vi "CaseSelect.vi"(11 "Owning VI Details":T5) -> ()   [LabVIEW 2020]
uses:
  Controls/btn-back-36x36.ctl
  Controls/btn-forward-36x36.ctl
  Controls/btn-clear-history-36x36.ctl
  Controls/btn-refresh-36x36.ctl
  <vilib>/event_ctls.llb/lveventtype.ctl
  JKI State Machine API/source/JKI SM/JKI SM.lvclass
  <vilib>/Utility/miscctls.llb/LVRectTypeDef.ctl
  JKI State Machine API/source/JKI SM/JKI SM.lvclass/JKI SM.ctl
  <vilib>/Utility/traverseref.llb/TRef TravTarget.ctl
  <vilib>/addons/_JKI Toolkits/State Machine/_JKI_lib_State_Machine.llb/Select State(s)_bool__jki_lib_state_machine.vi
  48b0ad3e-4641-4b59-aa41-8f6ed30ff61c.vi
  <userlib>/_OpenG.lib/comparison/comparison.llb/String Changed__ogtk.vi
  <userlib>/_OpenG.lib/comparison/comparison.llb/1D String Array Changed__ogtk.vi
  <userlib>/_OpenG.lib/file/file.llb/Build Path - File Names Array - path__ogtk.vi
  <vilib>/regexp/Match Regular Expression.xnode
  <userlib>/_OpenG.lib/comparison/comparison.llb/openg_comparison__ogtk.lvlib
  <userlib>/_OpenG.lib/time/time.llb/openg_time.lvlib
  <userlib>/_OpenG.lib/file/file.llb/openg_file.lvlib
panel:
  in  "Refresh":T1
  in  "Clear History":T2
  in  "Forward":T3
  in  "Back":T4
  in  "Search Icon":bool
  in  "Clear Search":bool
  in  "Search":string
  in  "Add macro":bool
  in  "Tree":string(tree) caption="Cases"
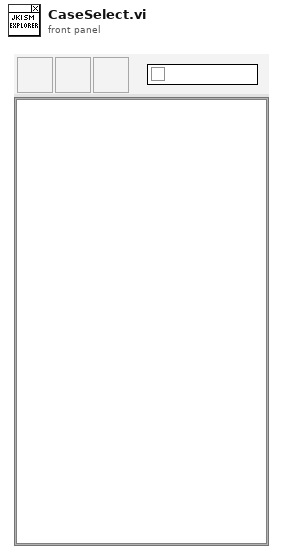
[diagram p1: front panel]
types:
  T1 = typedef "btn-refresh-36x36.ctl" = bool
  T2 = typedef "btn-clear-history-36x36.ctl" = bool
  T3 = typedef "btn-forward-36x36.ctl" = bool
  T4 = typedef "btn-back-36x36.ctl" = bool
  T5 = cluster{"App.ContextName":string, "VI.Name":string, "Object UID":i32}
  T6 = enum32{"Invalid", "Standard", "Closed", "Hidden", "Minimized", "Maximized"}
  T7 = typedef "lveventtype.ctl" = enum32{"Null", "Timeout", "Annotation Menu Selection", "Annotation Menu Selection?", "App Instance Close", "App Instance Close?", "Autoscale Range Change", "Bookmark Info Change", "Cell Edit", "Cell Edit?", "Cursor Grab", "Cursor Grab?", "Cursor Menu Selection", "Cursor Menu Selection?", "Cursor Move", "Cursor Release", "Data Change", "Direction Change", "Display State Change", "Drag Ended", "Drag Enter", "Drag Leave", "Drag Over", "Drag Source Update", "Drag Starting", "Drag Starting?", "Drop", "Exec State Change", "Key Down", "Key Down?", "Key Repeat", "Key Repeat?", "Key Up", "Listbox Double Click", "Menu Activation?", "Menu Selection (App)", "Menu Selection? (App)", "Menu Selection (User)", "Mouse Down", "Mouse Down?", "Mouse Enter", "Mouse Leave", "Mouse Move", "Mouse Up", "Mouse Wheel", "NI Security User Change (App)", "Pane Size", "Panel Close", "Panel Close?", "Panel Resize", "Plot Attribute Change", "Scale Range Change", "Shortcut Menu Activation?", "Shortcut Menu Selection (App)", "Shortcut Menu Selection? (App)", "Shortcut Menu Selection (User)", "Tree Double Click", "Tree Drag", "Tree Drag?", "Tree Drop", "Tree Drop?", "Tree Item Close", "Tree Item Close?", "Tree Item Open", "Tree Item Open?", "User Event", "Value Change"}
  T8 = enum32{"invalid app kind", "Development System", "Run Time System", "Student Edition", "Embedded LabVIEW", "Evaluation", "Custom"}
  T9 = typedef "TRef TravTarget.ctl" = enum16{"FP", "BD", "Other"}
  T10 = typedef "LVPoint32TypeDef.ctl" = cluster{"Horizontal":i32, "Vertical":i32}
  T11 = typedef "LVNodeAndColumnTypeDef.ctl" = cluster{"Node":string, "Column":i32}
  T12 = typedef "LVRectTypeDef.ctl" = cluster{"Left":i16, "Top":i16, "Right":i16, "Bottom":i16}
  T13 = cluster{"OpenCategoryFrames":refnum<vi>[], "Frames[]":refnum<vi>[], "Core":cluster{"Current VI Reference":refnum<vi>, "Close Panel on Exit?":bool}, "Indent?":bool, "InBounds":bool, "Activating":bool, "FrameNames":string[], "tag":string, "Top Row Tag":string, "TreeSectHdrs":string, "SectHdr":string, "CaseStrVIName":string, "TempString":string, "DisplayedItems":i32, "SelectedCase":u32, "Display:Primary Workspace":T12, "Tree":refnum<vi>, "StructRef":refnum<vi>, "CaseStrVI Ref":refnum<vi>, "Ctrl?":bool, "NavHist":refnum<vi>[], "NavIndex":i32, "Undo Transaction":bool, "Top Row Index":i32, "JKI SM":refnum<class "JKI SM.lvclass">, "Num Event Frames":i32, "Error During Startup":bool}
  T14 = cluster{"Current VI Reference":refnum<vi>, "Close Panel on Exit?":bool}
  T15 = enum8{"Enabled", "Disabled", "Disabled and Grayed Out"}
  T16 = enum32{"Bad", "Idle", "Run top level", "Running"}
  T17 = typedef "StructureTypes.ctl" = enum16{"CaseStructure", "EventStructure"}
  T18 = cluster{"StringConstant":refnum<vi>, "Structure":string, "Frame Name":string, "State Call":string, "UID":dbl}[]
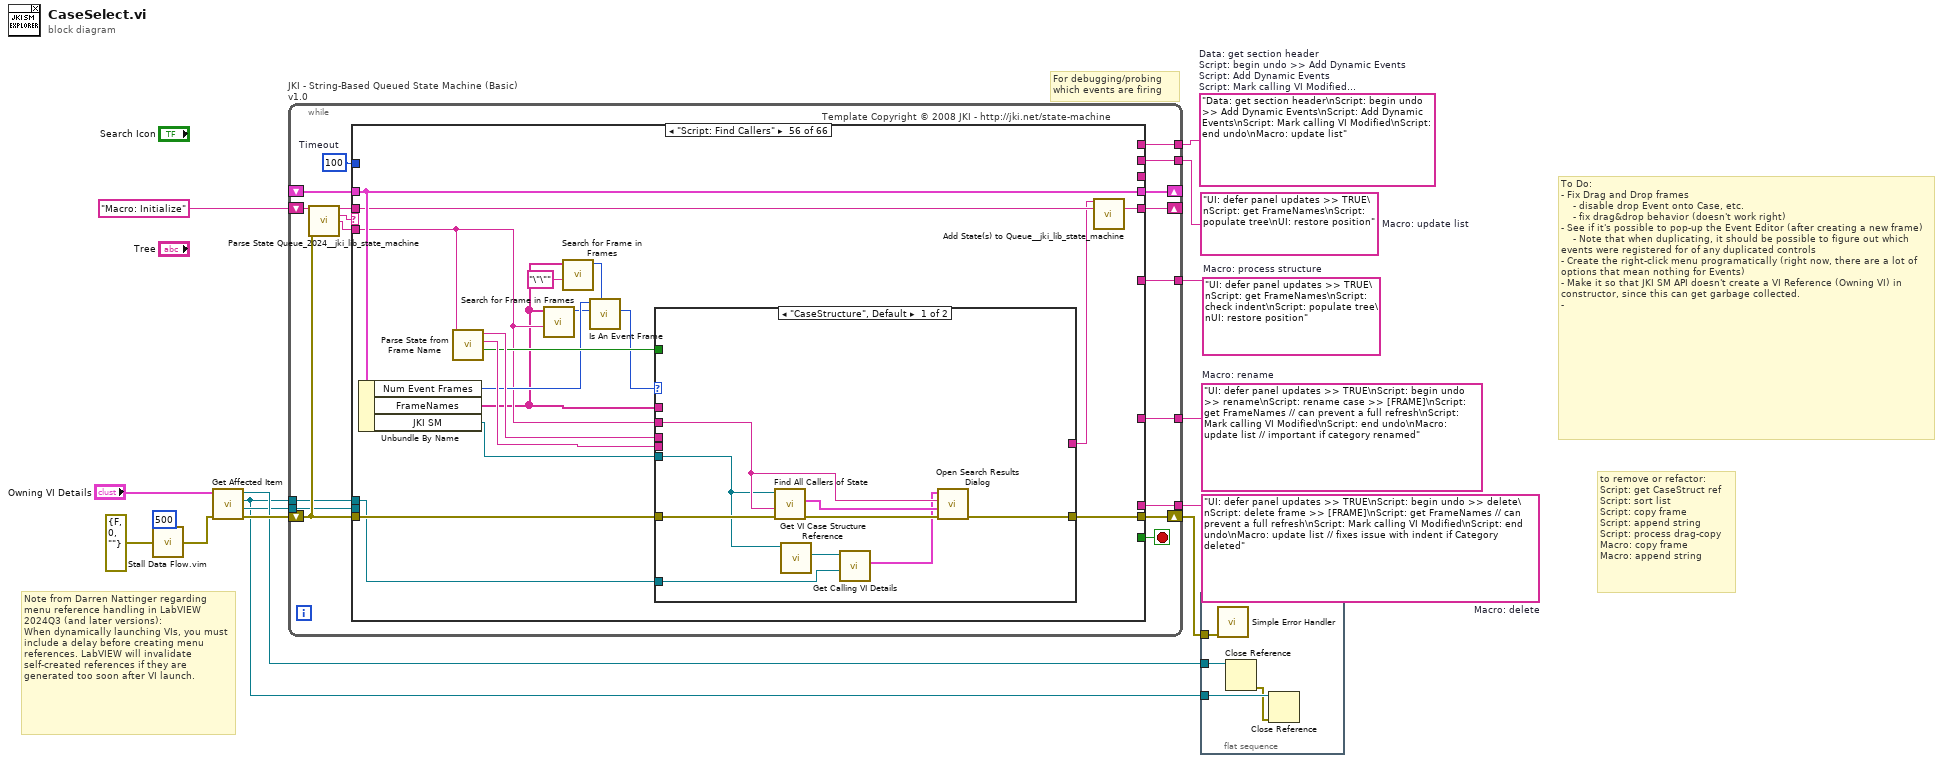
[diagram p0: block diagram]
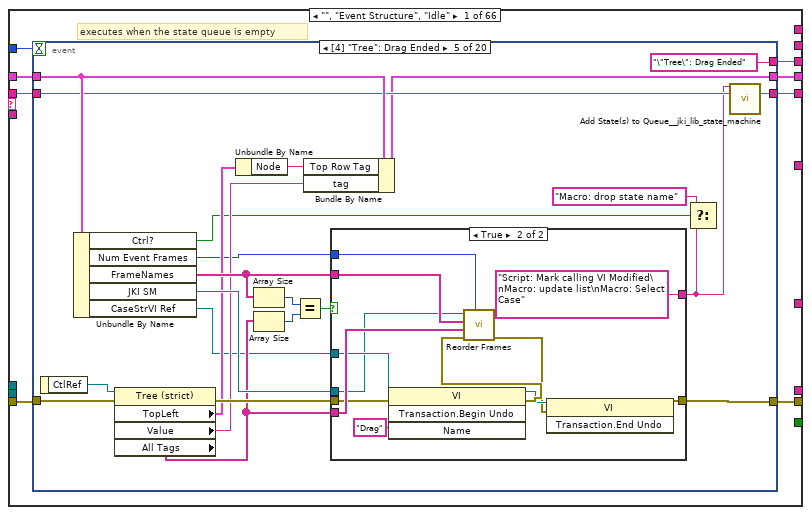
[diagram p2: hidden frame]
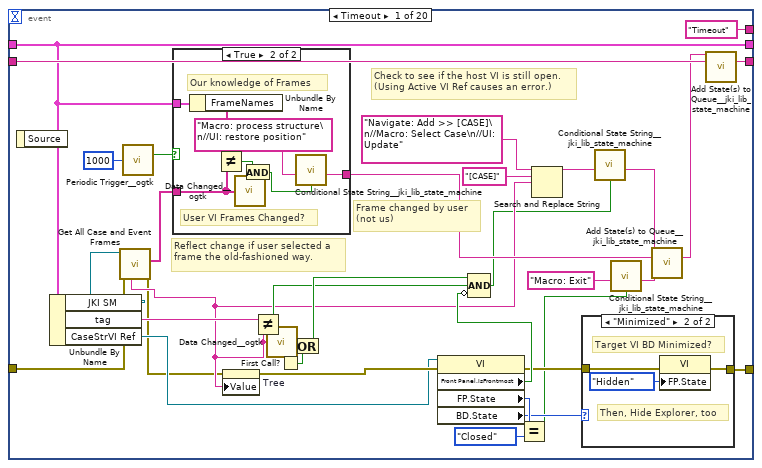
[diagram p3: hidden frame]
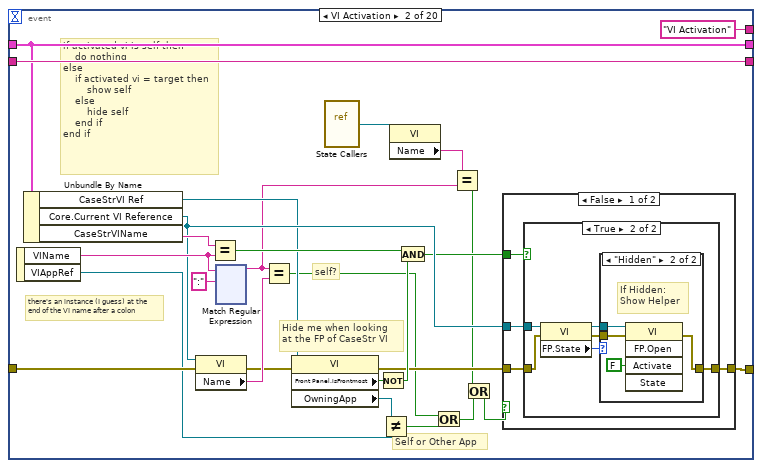
[diagram p6: hidden frame]
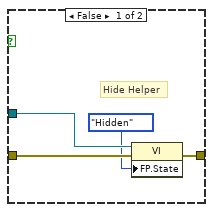
[diagram p7: hidden frame]
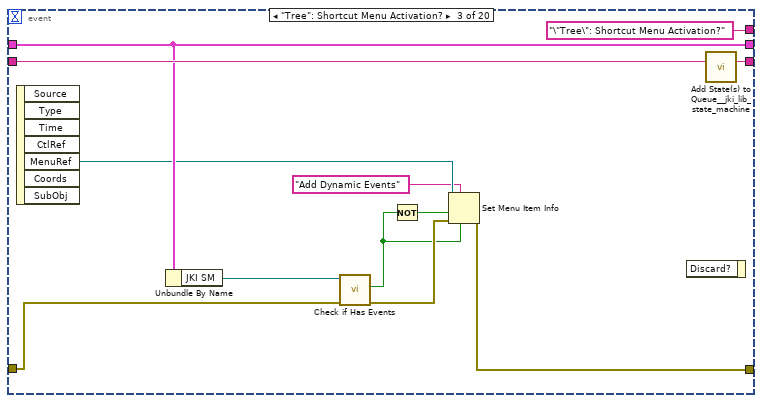
[diagram p10: hidden frame]
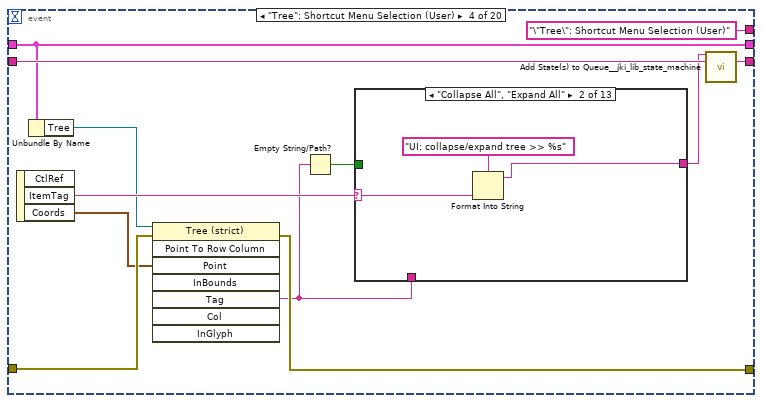
[diagram p11: hidden frame]
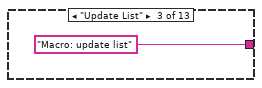
[diagram p13: hidden frame]
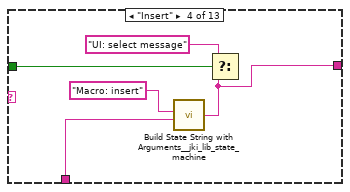
[diagram p14: hidden frame]
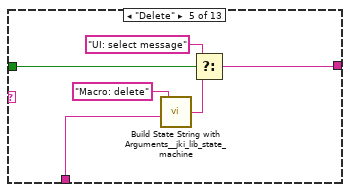
[diagram p15: hidden frame]
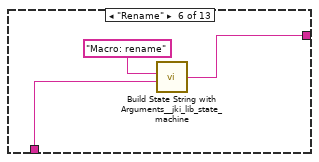
[diagram p16: hidden frame]
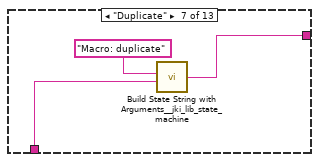
[diagram p17: hidden frame]
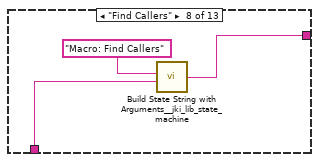
[diagram p18: hidden frame]
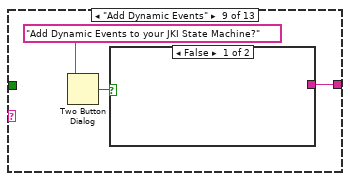
[diagram p19: hidden frame]
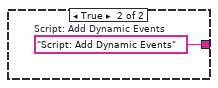
[diagram p20: hidden frame]
diagram:
  w9 = "Data: get section header\nScript: begin undo >> Add Dynamic Events\nScript: Add Dynamic Events\nScript: Mark calling VI Modified\nScript: end undo\nMacro: update list"  # Data: get section header Script: begin undo >> Add Dynamic Events Script: Add Dynamic Events Script: Mark calling VI Modified Script: end undo Macro: update list
  w10 = "UI: defer panel updates >> TRUE\nScript: get FrameNames\nScript: populate tree\nUI: restore position"  # Macro: update list
  w12 = "UI: defer panel updates >> TRUE\nScript: begin undo >> delete\nScript: delete frame >> [FRAME]\nScript: get FrameNames // can prevent a full refresh\nScript: Mark calling VI Modified\nScript: end undo\nMacro: update list // fixes issue with indent if Category deleted"  # Macro: delete
  w13 = "UI: defer panel updates >> TRUE\nScript: begin undo >> rename\nScript: rename case >> [FRAME]\nScript: get FrameNames // can prevent a full refresh\nScript: Mark calling VI Modified\nScript: end undo\nMacro: update list // important if category renamed"  # Macro: rename
  w14 = "UI: defer panel updates >> TRUE\nScript: get FrameNames\nScript: check indent\nScript: populate tree\nUI: restore position"  # Macro: process structure
  # "Note from Darren Nattinger regarding menu reference handling in LabVIEW 2024Q3 (and later versions):\nWhen dynamically launching VIs, you must include a delay before creating menu references. LabVIEW will invalidate self-created references if they are generated too soon after VI launch."
  # "to remove or refactor:\nScript: get CaseStruct ref\nScript: sort list\nScript: copy frame\nScript: append string\nScript: process drag-copy\nMacro: copy frame\nMacro: append string"
  # "For debugging/probing which events are firing"
  # "To Do:\n- Fix Drag and Drop frames\n    - disable drop Event onto Case, etc.\n    - fix drag&drop behavior (doesn't work right)\n- See if it's possible to pop-up the Event Editor (after creating a new frame)\n    - Note that when duplicating, it should be possible to figure out which events were registered for of any duplicated controls\n- Create the right-click menu programatically (right now, there are a lot of options that mean nothing for Events)\n- Make it so that JKI SM API doesn't create a VI Reference (Owning VI) in constructor, since this can get garbage collected.\n-"
  n1 = call "Stall Data Flow.vim"("value in"=errorcluster {"status"=FALSE, "code"=0, "source"=""} ("error in (no error)"), "milliseconds to wait"=u32 500) -> ("value out"=w5:errorcluster)  [unwired: 1 out]
  n2 = call "Get Affected Item.vi"("error in (no error)"=w5, "Owning VI Details"="Owning VI Details") -> ("error out"=w7:errorcluster, "GObject"=w2:refnum<vi>, "Owning VI"=w1:refnum<vi>, "Application"=w6:refnum<vi>)  [unwired: 6 in]
  n3 = while "JKI - String-Based Queued State Machine (Basic) v1.0" {
    shift-right: [w30] -> _
    shift-left: _ -> [w29]
    shift-right: [w33] -> w11
    shift-left: w7 -> [w21]
    shift-right: [w32] -> _
    shift-left: "Macro: Initialize" -> [w22]
    tunnel: w14 -> [w27]
    tunnel: w13 -> [w26]
    tunnel: w12 -> [w25]
    tunnel: w10 -> [w24]
    tunnel: w9 -> [w23]
    tunnel: w2 -> [w17]
    tunnel: w1 -> [w16]
    stop <- w31 stop-if-true
    w28 = 100  # Timeout
    # "Template Copyright © 2008 JKI - http://jki.net/state-machine"
    n4 = call <vilib>:"Parse State Queue_2024__jki_lib_state_machine.vi"("State Queue"=w22, "Error In (no error)"=w21) -> ("Remaining States"=w18:string, "Current State"=w19:string, "Arguments"=w20:string)  [unwired: 11 in]
    n5 = case shown="\"Script: Find Callers\"" w19 {
      selector: w19 -> [_ _ w578 _ _ _ _ _ _ _ _ _ _ _ _ _ _ _ _ _ _ _ _ _ _ _ _ _ _ _ _ _ _ _ _ _ _ _ _ _ _ _ _ _ _ _ _ _ _ _ _ _ _ _ _ _ _ _ _ _ _ _ _ _ _ _]
      tunnel: w18 -> [w41 w574 w577 w587 w606 _ w632 w636 w657 w698 w715 w728 w731 w739 w755 w757 w799 w809 w827 w852 w881 w893 w895 w902 w905 w913 w923 w942 w945 w951 w955 w966 w974 w979 w988 w992 w997 w1007 w1014 w1015 w1028 w1045 w1046 w1059 w1073 w1093 w1094 w1133 w1188 w1209 w1214 w1223 w1305 w1351 w1398 w1456 w1485 w1511 w1546 w1569 w1578 w1588 w1596 w1611 w1661 w1670]
      tunnel: w20 -> [_ _ _ _ _ w617 _ _ _ _ _ _ _ _ _ w756 _ w812 _ w854 _ _ _ _ _ w908 w919 w938 _ _ _ w959 w971 _ w985 _ _ w1004 _ _ w1018 _ _ w1056 _ _ _ _ _ _ _ w1217 w1299 w1340 w1390 w1445 w1478 _ w1535 _ _ _ _ _ _ _]
      tunnel: w29 -> [w39 w575 w580 w590 w607 w624 w635 w637 _ w697 w713 w729 w732 w740 w753 w759 w798 w814 w831 w850 w880 w892 w896 w899 w906 w914 w924 w935 w946 w949 w957 w960 w975 w980 w989 w994 w999 w1009 w1011 w1016 w1026 w1042 w1047 w1057 w1072 w1091 w1102 w1116 w1187 w1208 w1213 w1225 w1308 w1344 w1400 w1458 w1486 w1521 w1551 w1570 w1577 w1587 w1595 w1621 w1660 w1669]
      tunnel: [w38 w576 w582 w596 w608 w625 w634 w638 w641 w699 w714 w722 w733 w738 w754 w760 w796 w815 w832 w856 w879 w894 w897 w900 w907 w915 w917 w937 w947 w952 w956 w962 w969 w977 w983 w993 w998 w1008 w1012 w1017 w1022 w1037 w1048 w1058 w1069 w1087 w1095 w1128 w1186 w1207 w1211 w1219 w1307 w1352 w1399 w1457 w1475 w1515 w1537 w1568 w1574 w1584 w1592 w1614 w1655 w1665] -> w33
      tunnel: w21 -> [w37 w576 w581 w596 w608 w619 w634 w638 w651 w699 w714 w727 w733 w738 w754 w761 w797 w816 w833 w855 w882 w894 w897 w900 w907 w915 w918 w933 w947 w952 w956 w963 w970 w977 w984 w993 w998 w1008 w1012 w1017 w1020 w1038 w1048 w1052 w1070 w1078 w1096 w1134 w1177 w1206 w1212 w1226 w1297 w1349 w1394 w1452 w1476 w1519 w1536 w1568 w1576 w1586 w1594 w1620 w1657 w1668]
      tunnel: [w40 w574 w577 w587 w606 w621 w632 w636 w657 w698 w715 w728 w731 w739 w755 w757 w799 w808 w826 w851 w881 w893 w895 w901 w904 w912 w922 w941 w944 w950 w954 w965 w973 w978 w987 w991 w996 w1006 w1013 w1015 w1028 w1045 w1046 w1059 w1073 w1092 w1094 w1133 w1188 w1209 w1214 w1222 w1304 w1351 w1397 w1455 w1484 w1510 w1545 w1569 w1578 w1588 w1596 w1610 w1661 w1670] -> w32
      tunnel: [_ _ _ _ _ _ TRUE _ _ _ _ _ _ _ _ _ _ _ _ _ _ _ _ _ _ _ _ _ _ _ _ _ _ _ _ _ _ _ _ _ _ _ _ _ _ _ _ _ _ _ _ _ _ _ _ _ _ _ _ _ _ _ _ _ _ _] -> w31
      tunnel: [w36 w575 w580 w597 w607 w624 w635 w637 w679 w696 w709 w729 w732 w740 w753 w759 w798 w814 w828 w849 w880 w892 w896 w899 w906 w914 w924 w935 w946 w949 w957 w960 w975 w980 w989 w994 w999 w1009 w1011 w1016 w1027 w1041 w1047 w1055 w1071 w1090 w1101 w1132 w1183 w1208 w1213 w1225 w1308 w1343 w1400 w1458 w1486 w1509 w1541 w1570 w1573 w1587 w1591 w1621 w1660 w1669] -> w30
      tunnel: w28 -> [w35 _ _ _ _ _ _ _ _ _ _ _ _ _ _ _ _ _ _ _ _ _ _ _ _ _ _ _ _ _ _ _ _ _ _ _ _ _ _ _ _ _ _ _ _ _ _ _ _ _ _ _ _ _ _ _ _ _ _ _ _ _ _ _ _ _]
      tunnel: w27 -> [_ _ _ _ _ _ _ _ _ _ _ _ _ _ _ _ _ _ _ _ _ _ _ _ w903 _ _ _ _ _ _ _ _ _ _ _ _ _ _ _ _ _ _ _ _ _ _ _ _ _ _ _ _ _ _ _ _ _ _ _ _ _ _ _ _ _]
      tunnel: w26 -> [_ _ _ _ _ _ _ _ _ _ _ _ _ _ _ _ _ _ _ _ _ _ _ _ _ _ _ _ _ _ _ w958 _ _ _ _ _ _ _ _ _ _ _ _ _ _ _ _ _ _ _ _ _ _ _ _ _ _ _ _ _ _ _ _ _ _]
      tunnel: w25 -> [_ _ _ _ _ _ _ _ _ _ _ _ _ _ _ _ _ _ _ _ _ _ _ _ _ _ w916 _ _ _ _ _ _ _ _ _ _ _ _ _ _ _ _ _ _ _ _ _ _ _ _ _ _ _ _ _ _ _ _ _ _ _ _ _ _ _]
      tunnel: w24 -> [_ _ _ _ _ _ _ _ _ _ _ _ _ _ _ _ _ _ _ _ _ _ _ _ _ _ _ _ w943 _ _ _ _ _ _ _ _ _ _ _ _ _ _ _ _ _ _ _ _ _ _ _ _ _ _ _ _ _ _ _ _ _ _ _ _ _]
      tunnel: w23 -> [_ _ _ _ _ _ _ _ _ _ _ _ _ _ _ _ _ _ _ _ _ _ _ _ _ _ _ _ _ _ _ _ _ w976 _ _ _ _ _ _ _ _ _ _ _ _ _ _ _ _ _ _ _ _ _ _ _ _ _ _ _ _ _ _ _ _]
      tunnel: [w34 _ _ _ _ _ _ _ _ _ _ _ _ _ _ _ _ _ _ _ _ _ _ _ _ _ _ _ _ _ _ _ _ _ _ _ _ _ _ _ _ _ _ _ _ _ _ _ _ _ _ _ _ _ _ _ _ _ _ _ _ _ _ _ _ _] -> _
      tunnel: w17 -> [_ _ _ _ _ _ _ _ w640 _ _ _ _ _ _ _ _ _ _ _ _ _ _ _ _ _ _ _ _ _ _ _ _ _ _ _ _ _ _ _ _ _ _ _ _ _ _ _ _ _ _ _ _ _ _ _ _ _ _ _ _ _ _ _ _ _]
      tunnel: w16 -> [_ _ _ _ _ _ _ _ w639 _ _ _ _ _ _ _ _ _ _ _ _ _ _ _ _ _ _ _ _ _ _ _ _ _ _ _ _ _ _ _ _ _ _ _ _ _ _ _ _ _ _ _ _ _ _ w1441 _ _ _ _ _ _ _ _ _ _]
      frame "", "Event Structure", "Idle" {
        # "executes when the state queue is empty"
        n6 = event shown="[4] \"Tree\": Drag Ended" {
          selector: _ -> [_ _ _ _ _ _ _ _ _ _ _ _ _ _ _ _ _ _ _ _]
          dyn-events: _ -> [_ _ _ _ _ _ _ _ _ _ _ _ _ _ _ _ _ _ _ _]
          timeout: w35 -> [_ _ _ _ _ _ _ _ _ _ _ _ _ _ _ _ _ _ _ _]
          tunnel: w41 -> [w75 w114 w257 w267 w319 w346 w356 w363 w397 w442 w458 w494 w497 w506 w515 w536 w555 w559 w566 w573]
          tunnel: [w74 w114 w256 w266 w318 w345 w356 w362 w396 w442 w457 w494 w496 w505 w514 w535 w554 w560 w566 w572] -> w40
          tunnel: w39 -> [w57 w112 w255 w264 w321 w347 w355 w360 w391 w439 w459 w492 w500 w509 w518 w548 w552 w561 w564 w570]
          tunnel: [w48 w110 w250 w260 w308 w343 w351 w364 w394 w435 w460 w493 w499 w508 w517 w527 w556 w562 w563 w571] -> w38
          tunnel: w37 -> [w53 w102 w254 w269 w323 w343 w352 w365 w394 w436 w460 w493 w499 w508 w517 w524 w556 w562 w563 w571]
          tunnel: [w57 w112 w255 w264 w312 w344 w350 w360 w390 w439 w455 w492 w500 w509 w518 w549 w552 w561 w564 w570] -> w36
          tunnel: ["Timeout" ("State(s) in Front (\"\")") "VI Activation" ("State(s) in Front (\"\")") "\"Tree\": Shortcut Menu Activation?" ("State(s) in Front (\"\")") "\"Tree\": Shortcut Menu Selection (User)" ("State(s) in Front (\"\")") "\"Tree\": Drag Ended" ("State(s) in Front (\"\")") "\"Tree\": Value Change" ("State(s) in Front (\"\")") "\"Tree\": Mouse Down" ("State(s) in Front (\"\")") "\"Tree\": Mouse Up" ("State(s) in Front (\"\")") "\"Tree\": Item Close" ("State(s) in Front (\"\")") "\"Tree\": Mouse Move" ("State(s) in Front (\"\")") "Key Down?" ("State(s) in Front (\"\")") "Mouse Leave" ("State(s) in Front (\"\")") "Panel Resize" ("State(s) in Front (\"\")") "\"Search\": Value Change" ("State(s) in Front (\"\")") "\"Clear Search\": Value Change" ("State(s) in Front (\"\")") "\"Back\", \"Forward\": Value Change" ("State(s) in Front (\"\")") "\"Clear History\": Value Change" ("State(s) in Front (\"\")") "\"Refresh\": Value Change" ("State(s) in Front (\"\")") "\"Add macro\": Value Change" ("State(s) in Front (\"\")") "Panel Close?" ("State(s) in Front (\"\")")] -> w34
          event Timeout {
            # "Frame changed by user\n(not us)"
            # "Reflect change if user selected a frame the old-fashioned way."
            # "Check to see if the host VI is still open.\n(Using Active VI Ref causes an error.)"
            n7 = event-data() -> ()  [unwired: 2 out]
            n8 = Unbundle By Name(w57) -> ("JKI SM"=w56:refnum<class "JKI SM.lvclass">, "tag"=w70:string, "CaseStrVI Ref"=w60:refnum<vi>)
            n9 = call "Get All Case and Event Frames.vi"("error in (no error)"=w53, "JKI SM in"=w56) -> ("error out"=w52:errorcluster, "Frame Names"=w55:string[], "Visible Frame Name"=w54:string)  [unwired: 1 in, 6 out]
            n10 = call <userlib>:"Periodic Trigger__ogtk.vi"("time (ms)"=u32 1000) -> ("Triggered"=w62:bool)  [unwired: 12 in, 2 out]
            n11 = case shown="True" w62 {
              tunnel: [_ w80] -> w61
              tunnel: w57 -> [_ w87]
              tunnel: w55 -> [_ w83]
              frame False {
              }
              frame True {
                # "Our knowledge of Frames"
                # "User VI Frames Changed?"
                n12 = Unbundle By Name(w87) -> ("FrameNames"=w86:string[])
                n13 = Not Equal?(x=w86, y=w83) -> (x != y?=w85:bool)
                n14 = call-poly <userlib>:"Data Changed__ogtk.vi"("1D String Array"=w83) -> ("Changed"=w84:bool)
                n15 = And(x=w85, y=w84) -> (x .and. y?=w81:bool)
                n16 = call <vilib>:"Conditional State String__jki_lib_state_machine.vi"("Do State(s)?"=w81, "State"="Macro: process structure\n//UI: restore position") -> ("State Out"=w80:string)  [unwired: 7 in]
              }
            }
            n17 = property on="Tree" class="Tree (strict)"(error in=w52, "Value"=w54) -> (error out=w71:errorcluster)  [unwired: 1 in, 1 out]
            n18 = Not Equal?(x=w70, y=w54) -> (x != y?=w58:bool)
            n19 = call-poly <userlib>:"Data Changed__ogtk.vi"("String"=w54) -> ("Changed"=w65:bool)
            n20 = First Call?() -> (First Call?: T/F=w66:bool)
            n21 = Or(x=w65, y=w66) -> (x .or. y?=w64:bool)
            n22 = property class="VI"(reference=w60, error in=w71) -> (error out=w49:errorcluster, "Front Panel.IsFrontmost"=w59:bool, "FP.State"=w73:T6, "BD.State"=w50:T6)  [unwired: 1 out]
            n23 = Compound Arithmetic op=AND(w64, w58, invert w59) -> (w46:bool)
            n24 = Equal?(x=w73, y=T6."Closed" ("Front Panel Window:State")) -> (x = y?=w43:bool)
            n25 = Search and Replace String(input string="Navigate: Add >> [CASE]\n//Macro: Select Case\n//UI: Update" ("State(s) in Front (\"\")"), search string="[CASE]", replace string=w54) -> (result string=w47:string)  [unwired: 5 in, 3 out]
            n26 = case shown="\"Minimized\"" w50 {
              tunnel: w49 -> [w76 w79]
              tunnel: [w76 w78] -> w48
              frame Default {
              }
              frame "Minimized" {
                # "Then, Hide Explorer, too"
                # "Target VI BD Minimized?"
                n27 = property class="VI"(error in=w79, "FP.State"=T6."Hidden" ("Front Panel Window:State")) -> (error out=w78:errorcluster)  [unwired: 1 in, 1 out]
              }
            }
            n28 = call <vilib>:"Conditional State String__jki_lib_state_machine.vi"("Do State(s)?"=w46, "State"=w47) -> ("State Out"=w45:string)  [unwired: 7 in]
            n29 = call <vilib>:"Conditional State String__jki_lib_state_machine.vi"("Do State(s)?"=w43, "State"="Macro: Exit") -> ("State Out"=w42:string)  [unwired: 7 in]
            n30 = call <vilib>:"Add State(s) to Queue__jki_lib_state_machine.vi"("State(s) in Front (\"\")"=w45, "State(s) in (\"\")"=w61, "State(s) at Back (\"\")"=w42) -> ("States Out"=w67:string)  [unwired: 12 out]
            n31 = call <vilib>:"Add State(s) to Queue__jki_lib_state_machine.vi"("State(s) in Front (\"\")"=w67, "State(s) in (\"\")"=w75) -> ("States Out"=w74:string)  [unwired: 1 in, 12 out]
          }
          event VI Activation {
            # "Self or Other App"
            # "self?"
            # "Hide me when looking\nat the FP of CaseStr VI"
            # "there's an instance (I guess) at the\nend of the VI name after a colon"
            # "if activated vi is self then\n    do nothing\nelse\n    if activated vi = target then\n        show self\n    else\n        hide self\n    end if\nend if"
            n32 = event-data() -> ("VIName"=w107:string, "VIAppRef"=w97:refnum<vi>)  [unwired: 1 out]
            n33 = Unbundle By Name(w112) -> ("CaseStrVI Ref"=w100:refnum<vi>, "Core.Current VI Reference"=w106:refnum<vi>, "CaseStrVIName"=w113:string)
            n34 = property class="VI"(reference=w106, error in=w102) -> (error out=w101:errorcluster, "Name"=w108:string)  [unwired: 1 out]
            n35 = Equal?(x=w113, y=w107) -> (x = y?=w111:bool)
            n36 = xnode "Match Regular Expression"("input string"=w107, "regular expression"=":") -> ("before match"=w92:string)  [unwired: 3 in, 5 out]
            n37 = Equal?(x=w92, y=w108) -> (x = y?=w95:bool)
            n38 = property class="VI"(reference=w100, error in=w101) -> (error out=w103:errorcluster, "Front Panel.IsFrontmost"=w105:bool, "OwningApp"=w98:refnum<vi>)  [unwired: 1 out]
            n39 = vi-ref "State Callers.vi"() -> (w94:refnum<vi>)
            n40 = Not(x=w105) -> (.not. x?=w104:bool)
            n41 = Not Equal?(x=w98, y=w97) -> (x != y?=w96:bool)
            n42 = property class="VI"(reference=w94) -> ("Name"=w93:string)  [unwired: 1 in, 2 out]
            n43 = And(x=w111, y=w104) -> (x .and. y?=w99:bool)
            n44 = Or(x=w95, y=w96) -> (x .or. y?=w90:bool)
            n45 = Equal?(x=w93, y=w92) -> (x = y?=w91:bool)
            n46 = Or(x=w91, y=w90) -> (x .or. y?=w89:bool)
            n47 = case shown="False" w89 {
              tunnel: w103 -> [w118 w134]
              tunnel: [w116 w134] -> w110
              tunnel: w106 -> [w117 _]
              tunnel: w99 -> [w115 _]
              frame False {
                n48 = case shown="True" w115 {
                  tunnel: w118 -> [w122 w127]
                  tunnel: w117 -> [w121 w128]
                  tunnel: [w120 w125] -> w116
                  frame False {
                    # "Hide Helper"
                    n49 = property class="VI"(reference=w121, error in=w122, "FP.State"=T6."Hidden" ("Front Panel Window:State")) -> (error out=w120:errorcluster)  [unwired: 1 out]
                  }
                  frame True {
                    n50 = property class="VI"(reference=w128, error in=w127) -> (reference out=w124:refnum<vi>, error out=w123:errorcluster, "FP.State"=w126:T6)
                    n51 = case shown="\"Hidden\"" w126 {
                      tunnel: [w129 w133] -> w125
                      tunnel: w124 -> [_ w132]
                      tunnel: w123 -> [w129 w131]
                      frame Default {
                      }
                      frame "Hidden" {
                        # "If Hidden:\nShow Helper"
                        n52 = invoke class="VI" method="FP.Open"(reference=w132, error in=w131, "Activate"=FALSE ("Activate?")) -> (error out=w133:errorcluster)  [unwired: 2 in, 4 out]
                      }
                    }
                  }
                }
              }
              frame True {
              }
            }
          }
          event "Tree": Shortcut Menu Activation? {
            n53 = event-data() -> ("MenuRef"=w252:refnum<k9>)  [unwired: 7 out]
            n54 = Unbundle By Name(w255) -> ("JKI SM"=w247:refnum<class "JKI SM.lvclass">)
            n55 = call "Check if Has Events.vi"("error in (no error)"=w254, "JKI SM in"=w247) -> ("error out"=w251:errorcluster, "Has Dyanamic Events?"=w249:bool)  [unwired: 7 in, 1 out]
            n56 = Not(x=w249) -> (.not. x?=w253:bool)
            n57 = Set Menu Item Info(6:w249, 7:"Add Dynamic Events" ("item name"), 8:w251, 9:w253, 11:w252) -> (0:w250:errorcluster)  [unwired: 2 in, 1 out]
            n58 = event-data() -> ()  [unwired: 2 in, 1 out]
            n59 = call <vilib>:"Add State(s) to Queue__jki_lib_state_machine.vi"("State(s) in (\"\")"=w257) -> ("States Out"=w256:string)  [unwired: 2 in, 12 out]
          }
          event "Tree": Shortcut Menu Selection (User) {
            n60 = event-data() -> ("ItemTag"=w268:string, "Coords"=w261:T10)  [unwired: 2 out]
            n61 = Unbundle By Name(w264) -> ("Tree"=w263:refnum<vi>)
            n62 = invoke class="Tree (strict)" method="Point To Row Column"(reference=w263, error in=w269, "Point"=w261) -> (error out=w260:errorcluster, "Tag"=w259:string)  [unwired: 5 in, 6 out]
            n63 = Empty String/Path?(string/path=w259) -> (empty?=w262:bool)
            n64 = case shown="\"Collapse All\", \"Expand All\"" w268 {
              selector: w268 -> [_ w271 _ _ _ _ _ _ _ _ _ _ _]
              tunnel: [_ w270 "Macro: update list" w274 w282 w285 w288 w291 w296 "Macro: sort list" _ w299 _] -> w265
              tunnel: w262 -> [_ _ _ w278 w284 _ _ _ _ _ _ _ _]
              tunnel: w259 -> [_ _ _ w275 w280 w287 w290 w293 _ _ _ _ w300]
              frame Default {
              }
              frame "Collapse All", "Expand All" {
                n65 = Format Into String(format string="UI: collapse/expand tree >> %s", w271) -> (resulting string=w270:string)  [unwired: 2 in, 1 out]
              }
              frame "Update List" {
              }
              frame "Insert" {
                n66 = call <vilib>:"Build State String with Arguments__jki_lib_state_machine.vi"("Arguments (\"\")"=w275, "State"="Macro: insert") -> ("State with Arguments"=w274:string)  [unwired: 4 in]
                n67 = Select(t="UI: select message", s=w278, f=w274) -> ()  [unwired: 1 out]
              }
              frame "Delete" {
                n68 = call <vilib>:"Build State String with Arguments__jki_lib_state_machine.vi"("Arguments (\"\")"=w280, "State"="Macro: delete") -> ("State with Arguments"=w279:string)  [unwired: 4 in]
                n69 = Select(t="UI: select message", s=w284, f=w279) -> (s? t:f=w282:string)
              }
              frame "Rename" {
                n70 = call <vilib>:"Build State String with Arguments__jki_lib_state_machine.vi"("Arguments (\"\")"=w287, "State"="Macro: rename") -> ("State with Arguments"=w285:string)  [unwired: 4 in]
              }
              frame "Duplicate" {
                n71 = call <vilib>:"Build State String with Arguments__jki_lib_state_machine.vi"("Arguments (\"\")"=w290, "State"="Macro: duplicate") -> ("State with Arguments"=w288:string)  [unwired: 4 in]
              }
              frame "Find Callers" {
                n72 = call <vilib>:"Build State String with Arguments__jki_lib_state_machine.vi"("Arguments (\"\")"=w293, "State"="Macro: Find Callers") -> ("State with Arguments"=w291:string)  [unwired: 4 in]
              }
              frame "Add Dynamic Events" {
                n73 = Two Button Dialog(message="Add Dynamic Events to your JKI State Machine?" ("format string")) -> (T button?=w295:bool)  [unwired: 2 in]
                n74 = case shown="False" w295 {
                  tunnel: [_ w297] -> w296
                  frame False {
                  }
                  frame True {
                    w297 = "Script: Add Dynamic Events"  # Script: Add Dynamic Events
                  }
                }
              }
              frame "Sort" {
              }
              frame "About" {
                n75 = call "About.vi"() -> ()  [unwired: 1 out]
              }
              frame "highlight" {
                w299 = "Script: highlight"  # Script: highlight
              }
              frame "Copy State Name to Clipboard" {
                n76 = call "Copy State Name to Clipboard.vi"("Tag"=w300) -> ()  [unwired: 11 in]
              }
            }
            n77 = call <vilib>:"Add State(s) to Queue__jki_lib_state_machine.vi"("State(s) in Front (\"\")"=w265, "State(s) in (\"\")"=w267) -> ("States Out"=w266:string)  [unwired: 1 in, 12 out]
          }
          event "Tree": Drag Ended {
            n78 = event-data() -> ("CtlRef"=w322:refnum<vi>)  [unwired: 1 out]
            n79 = Unbundle By Name(w321) -> ("Ctrl?"=w305:bool, "Num Event Frames"=w301:i32, "FrameNames"=w316:string[], "JKI SM"=w320:refnum<class "JKI SM.lvclass">, "CaseStrVI Ref"=w304:refnum<vi>)
            n80 = property class="Tree (strict)"(reference=w322, error in=w323) -> (error out=w317:errorcluster, "TopLeft"=w311:T11, "Value"=w307:string, "All Tags"=w309:string[])  [unwired: 1 out]
            n81 = Unbundle By Name(w311) -> ("Node"=w310:string)
            n82 = Array Size(array=w316) -> (size(s)=w314:i32)
            n83 = Array Size(array=w309) -> (size(s)=w315:i32)
            n84 = Equal?(x=w314, y=w315) -> (x = y?=w313:bool)
            n85 = Bundle By Name(cluster=w321, "Top Row Tag"=w310, "tag"=w307) -> (w312:T13)
            n86 = case shown="True" w313 {
              tunnel: w320 -> [_ w327]
              tunnel: w317 -> [w325 w335]
              tunnel: [w325 w331] -> w308
              tunnel: w316 -> [_ w337]
              tunnel: w309 -> [_ w336]
              tunnel: ["Macro: process drag-copy" ("message") "Script: Mark calling VI Modified\nMacro: update list\nMacro: Select Case" ("message")] -> w303
              tunnel: w304 -> [_ w328]
              tunnel: w301 -> [_ w326]
              frame False {
                # "There are more tags in the tree than\nthere are frames in the Case Structure.\nA drag/copy operation just occurred."
              }
              frame True {
                n87 = invoke class="VI" method="Transaction.Begin Undo"(reference=w328, error in=w335, "Name"="Drag") -> (reference out=w332:refnum<vi>, error out=w333:errorcluster)  [unwired: 1 in, 2 out]
                n88 = call "Reorder Frames.vi"("Num Event Frames"=w326, "error in (no error)"=w333, "Desired Frame Ordering"=w336, "Original Frame Ordering"=w337, "JKI SM in"=w327) -> ("error out"=w329:errorcluster)  [unwired: 6 in]
                n89 = invoke class="VI" method="Transaction.End Undo"(reference=w332, error in=w329) -> (error out=w331:errorcluster)  [unwired: 1 in, 2 out]
              }
            }
            n90 = Select(t="Macro: drop state name", s=w305, f=w303) -> ()  [unwired: 1 out]
            n91 = call <vilib>:"Add State(s) to Queue__jki_lib_state_machine.vi"("State(s) in Front (\"\")"=w303, "State(s) in (\"\")"=w319) -> ("States Out"=w318:string)  [unwired: 1 in, 12 out]
          }
          event "Tree": Value Change {
            n92 = event-data() -> ("NewVal"=w340:string)  [unwired: 1 out]
            n93 = Bundle By Name(cluster=w347, "tag"=w340) -> (w344:T13)
            n94 = Search and Replace String(input string="Navigate: Add >> [CASE]\nMacro: Select Case\nUI: Update" ("State(s) in Front (\"\")"), search string="[CASE]", replace string=w340) -> (result string=w339:string)  [unwired: 5 in, 3 out]
            n95 = call <vilib>:"Add State(s) to Queue__jki_lib_state_machine.vi"("State(s) in Front (\"\")"=w339, "State(s) in (\"\")"=w346) -> ("States Out"=w345:string)  [unwired: 1 in, 12 out]
          }
          event "Tree": Mouse Down {
            # "This makes a mouse click work\nonly if the click was in bounds."
            n96 = event-data() -> ("CtlRef"=w354:refnum<vi>, "Coords"=w353:T10)  [unwired: 4 out]
            n97 = invoke class="Tree (strict)" method="Point To Row Column"(reference=w354, error in=w352, "Point"=w353) -> (error out=w351:errorcluster, "InBounds"=w349:bool)  [unwired: 5 in, 6 out]
            n98 = Bundle By Name(cluster=w355, "InBounds"=w349) -> (w350:T13)
          }
          event "Tree": Mouse Up {
            n99 = event-data() -> ("Mods.Double Click"=w358:bool, "PlatMods.Ctrl"=w359:bool, "CtlRef"=w367:refnum<vi>, "Coords"=w366:T10)  [unwired: 1 out]
            n100 = case shown="True" w358 {
              tunnel: w367 -> [w379 _]
              tunnel: w366 -> [w378 _]
              tunnel: w365 -> [w377 w381]
              tunnel: [w376 w381] -> w364
              tunnel: [w375 "//Macro: append string"] -> w361
              tunnel: w360 -> [w374 _]
              tunnel: w359 -> [w373 _]
              frame False {
                n101 = invoke class="Tree (strict)" method="Point To Row Column"(reference=w379, error in=w377, "Point"=w378) -> (error out=w376:errorcluster, "InBounds"=w371:bool)  [unwired: 5 in, 6 out]
                n102 = Unbundle By Name(w374) -> ("InBounds"=w372:bool)
                n103 = Compound Arithmetic op=AND(invert w373, w372, w371) -> (w370:bool)
                n104 = Select(t="//Macro: Select Case", s=w370, f="") -> (s? t:f=w375:string)
              }
              frame True {
              }
            }
            n105 = call <vilib>:"Add State(s) to Queue__jki_lib_state_machine.vi"("State(s) in Front (\"\")"=w361, "State(s) in (\"\")"=w363) -> ("States Out"=w362:string)  [unwired: 1 in, 12 out]
          }
          event "Tree": Item Close; "Tree": event #0x1e {
            # "Find Frame by Name in our internal list"
            n106 = event-data() -> ("Type"=w388:T7, "Tag"=w392:string)  [unwired: 4 out]
            n107 = Unbundle By Name(w391) -> ("OpenCategoryFrames"=w386:refnum<vi>[], "Frames[]"=w387:refnum<vi>[], "FrameNames"=w393:string[])
            n108 = Equal?(x=w388, y=lveventtype."Tree Item Open" ("Type")) -> (x = y?=w382:bool)
            n109 = Search 1D Array(1D array=w393, element=w392) -> (index of element=w385:i32)  [unwired: 1 in]
            n110 = Greater Or Equal To 0?(x=w385) -> (x >= 0?=w384:bool)
            n111 = case shown="True" w384 {
              tunnel: w385 -> [_ w405]
              tunnel: w387 -> [_ w404]
              tunnel: w386 -> [w398 w401]
              tunnel: [w398 w402] -> w383
              tunnel: w382 -> [_ w399]
              frame False {
              }
              frame True {
                n112 = Index Array(array=w404, index=w405) -> (element=w400:refnum<vi>)
                n113 = Search 1D Array(1D array=w401, element=w400) -> (index of element=w403:i32)  [unwired: 1 in]
                n114 = case "Opening?" shown="True" w399 {
                  tunnel: w403 -> [w410 w415]
                  tunnel: [w408 w418] -> w402
                  tunnel: w401 -> [w407 w417]
                  tunnel: w400 -> [w406 w416]
                  frame True {
                    # "Opening Tree Item"
                    n115 = Greater Or Equal To 0?(x=w410) -> (x >= 0?=w409:bool)
                    n116 = case shown="True" w409 {
                      tunnel: [w412 w414] -> w408
                      tunnel: w407 -> [w413 w414]
                      tunnel: w406 -> [w411 _]
                      frame False {
                        # "Not Found\nAdd it"
                        n117 = Build Array (concatenate)(w413, w411) -> (w412:refnum<vi>[])
                      }
                      frame True {
                        # "Found\nIgnore"
                      }
                    }
                  }
                  frame False {
                    # "Closing Tree Item"
                    n118 = Greater Or Equal To 0?(x=w415) -> (x >= 0?=w419:bool)
                    n119 = case shown="True" w419 {
                      tunnel: [w420 w421] -> w418
                      tunnel: w417 -> [w420 w423]
                      tunnel: w416 -> [_ _]
                      tunnel: w415 -> [_ w422]
                      frame False {
                        # "Not Found\nIgnore"
                      }
                      frame True {
                        # "Found\nRemove it"
                        n120 = Delete From Array(array=w423, index=w422) -> (array with subset deleted=w421:refnum<vi>[])  [unwired: 1 in, 1 out]
                      }
                    }
                  }
                }
              }
            }
            n121 = Bundle By Name(cluster=w391, "OpenCategoryFrames"=w383) -> (w390:T13)
            n122 = call <vilib>:"Add State(s) to Queue__jki_lib_state_machine.vi"("State(s) in (\"\")"=w397) -> ("States Out"=w396:string)  [unwired: 2 in, 12 out]
          }
          event "Tree": Mouse Move {
            n123 = event-data() -> ("Coords"=w441:T10)  [unwired: 5 out]
            n124 = Unbundle By Name(w439) -> ("Num Event Frames"=w427:i32, "FrameNames"=w425:string[], "JKI SM"=w432:refnum<class "JKI SM.lvclass">)
            n125 = invoke on="Tree" class="Tree (strict)" method="Point To Row Column"(error in=w436, "Point"=w441) -> (error out=w437:errorcluster, "Tag"=w429:string)  [unwired: 6 in, 6 out]
            n126 = call "Search for Frame in Frames.vi"("Frame Name"=w429, "Frame Names"=w425) -> ("index of element"=w430:i32)  [unwired: 9 in]
            n127 = call "Search for Frame in Frames.vi"("Frame Name"="\"\"", "Frame Names"=w425) -> ("index of element"=w424:i32)  [unwired: 9 in]
            n128 = call "Is An Event Frame.vi"("Event Structure index"=w424, "index of element"=w430, "Num Event Frames"=w427) -> ("Event Frame?"=w428:bool)  [unwired: 7 in, 1 out]
            n129 = call-poly <userlib>:"Data Changed__ogtk.vi"("String"=w429) -> ("Changed"=w440:bool)
            n130 = call "Get Frame Documentation.vi"("Remove EOLs? (TRUE)"=TRUE, "Event Structure (F: Case Structure)"=w428, "error in (no error)"=w437, "State Name"=w429, "JKI SM in"=w432) -> ("error out"=w433:errorcluster, "Documentation"=w438:string)  [unwired: 4 in, 1 out]
            n131 = case shown="True" w440 {
              tunnel: w438 -> [_ w447]
              tunnel: w433 -> [w443 w446]
              tunnel: [w443 w445] -> w435
              tunnel: w429 -> [_ w444]
              frame False {
              }
              frame True {
                n132 = property on="Tree" class="Tree (strict)"(error in=w446, "Desc"=w447, "Caption.Text"=w444) -> (error out=w445:errorcluster)  [unwired: 1 in, 1 out]
              }
            }
          }
          event Key Down? {
            n133 = event-data() -> ("PlatMods.Shift"=w451:bool, "PlatMods.Ctrl"=w453:bool, "ScanCode"=w452:i16)  [unwired: 1 out]
            n134 = Bundle By Name(cluster=w459, "Ctrl?"=w453) -> (w455:T13)
            n135 = Unbundle By Name(w455) -> ("tag"=w454:string, "CaseStrVI Ref"=w450:refnum<vi>)
            n136 = case shown="44" w452 {
              tunnel: [_ w462 w466 w470 w475 _] -> w456
              tunnel: w454 -> [_ w464 w468 w472 w476 w485]
              tunnel: w453 -> [_ _ _ _ w474 w484]
              tunnel: w451 -> [_ _ _ _ _ w483]
              tunnel: w450 -> [_ _ _ _ _ w482]
              tunnel: [_ TRUE TRUE TRUE w473 w481] -> w449
              frame 0, Default {
              }
              frame 60 {
                # "F2"
                n137 = call <vilib>:"Build State String with Arguments__jki_lib_state_machine.vi"("Arguments (\"\")"=w464, "State"="Macro: rename") -> ("State with Arguments"=w462:string)  [unwired: 4 in]
              }
              frame 82 {
                n138 = call <vilib>:"Build State String with Arguments__jki_lib_state_machine.vi"("Arguments (\"\")"=w468, "State"="Macro: insert") -> ("State with Arguments"=w466:string)  [unwired: 4 in]
              }
              frame 83 {
                # "Delete"
                n139 = call <vilib>:"Build State String with Arguments__jki_lib_state_machine.vi"("Arguments (\"\")"=w472, "State"="Macro: delete") -> ("State with Arguments"=w470:string)  [unwired: 4 in]
              }
              frame 33 {
                # "Ctrl+F"
                n140 = case shown="True" w474 {
                  tunnel: w476 -> [_ w480]
                  tunnel: [_ w478] -> w475
                  tunnel: [_ TRUE] -> w473
                  frame False {
                  }
                  frame True {
                    n141 = call <vilib>:"Build State String with Arguments__jki_lib_state_machine.vi"("Arguments (\"\")"=w480, "State"="Macro: Find Callers") -> ("State with Arguments"=w478:string)  [unwired: 4 in]
                  }
                }
              }
              frame 44 {
                # "Z"
                n142 = case shown="True" w484 {
                  tunnel: w485 -> [_ _]
                  tunnel: w483 -> [_ w488]
                  tunnel: w482 -> [_ w487]
                  tunnel: [_ TRUE] -> w481
                  frame False {
                  }
                  frame True {
                    # "Ctrl+Z"
                    n143 = case shown="True" w488 {
                      tunnel: w487 -> [w489 w490]
                      frame False {
                        n144 = invoke class="VI" method="Transaction.Undo"(reference=w489) -> ()  [unwired: 2 in, 3 out]
                      }
                      frame True {
                        n145 = invoke class="VI" method="Transaction.Redo"(reference=w490) -> ()  [unwired: 2 in, 3 out]
                      }
                    }
                  }
                }
              }
            }
            n146 = event-data("Discard?"=w449) -> ()  [unwired: 1 in, 1 out]
            n147 = call <vilib>:"Add State(s) to Queue__jki_lib_state_machine.vi"("State(s) in Front (\"\")"=w456, "State(s) in (\"\")"=w458) -> ("States Out"=w457:string)  [unwired: 1 in, 12 out]
          }
          event Mouse Leave {
            n148 = event-data() -> ()  [unwired: 5 out]
          }
          event Panel Resize {
            n149 = event-data() -> ()  [unwired: 4 out]
            n150 = call <vilib>:"Add State(s) to Queue__jki_lib_state_machine.vi"("State(s) in Front (\"\")"="UI: show/hide scroll bar", "State(s) in (\"\")"=w497) -> ("States Out"=w496:string)  [unwired: 1 in, 12 out]
          }
          event "Search": Value Change {
            n151 = event-data() -> ("NewVal"=w504:string)  [unwired: 6 out]
            n152 = Empty String/Path?(string/path=w504) -> (empty?=w502:bool)
            n153 = Not(x=w502) -> (.not. x?=w503:bool)
            n154 = property on="Search Icon" class="Bool (strict)"("Visible"=w502) -> ()  [unwired: 2 in, 2 out]
            n155 = property on="Clear Search" class="Bool (strict)"("Visible"=w503) -> ()  [unwired: 2 in, 2 out]
            n156 = call <vilib>:"Add State(s) to Queue__jki_lib_state_machine.vi"("State(s) in Front (\"\")"="Macro: process structure", "State(s) in (\"\")"=w506) -> ("States Out"=w505:string)  [unwired: 1 in, 12 out]
          }
          event "Clear Search": Value Change {
            n157 = event-data() -> ()  [unwired: 7 out]
            n158 = property on="Clear Search" class="Bool (strict)"("Visible"=FALSE) -> ()  [unwired: 2 in, 2 out]
            n159 = property on="Search Icon" class="Bool (strict)"("Visible"=TRUE) -> ()  [unwired: 2 in, 2 out]
            n160 = local write "Search"("" ("Search")) -> ()
            n161 = call <vilib>:"Add State(s) to Queue__jki_lib_state_machine.vi"("State(s) in Front (\"\")"="Macro: process structure", "State(s) in (\"\")"=w515) -> ("States Out"=w514:string)  [unwired: 1 in, 12 out]
          }
          event Value Change {
            n162 = event-data() -> ()  [unwired: 7 out]
            n163 = Unbundle By Name(w548) -> ("NavIndex"=w537:i32, "NavHist"=w539:refnum<vi>[], "JKI SM"=w529:refnum<class "JKI SM.lvclass">)
            n164 = Decrement(x=w537) -> (x-1=w547:i32)
            n165 = Increment(x=w537) -> (x+1=w546:i32)
            n166 = call "Get All Case and Event Frames.vi"("error in (no error)"=w524, "JKI SM in"=w529) -> ("error out"=w523:errorcluster, "Frame Names"=w531:string[], "Frames[]"=w530:refnum<vi>[], "Num Event Frames"=w526:i32, "Event Frame Index"=w519:i32)  [unwired: 1 in, 4 out]
            n167 = Select(t=w547, s="Back", f=w546) -> (s? t:f=w543:i32)
            n168 = Array Size(array=w539) -> (size(s)=w545:i32)
            n169 = Decrement(x=w545) -> (x-1=w538:i32)
            n170 = In Range and Coerce(upper limit=w538, x=w543, lower limit=0) -> (coerced(x)=w540:i32, In Range?=w542:bool)
            n171 = Index Array(array=w539, index=w540) -> (element=w532:refnum<vi>)
            n172 = Search 1D Array(1D array=w530, element=w532) -> (index of element=w521:i32)  [unwired: 1 out]
            n173 = To Unsigned Long Integer(number=w521) -> (unsigned 32bit integer=w550:u32)
            n174 = call "Is An Event Frame.vi"("Event Structure index"=w519, "index of element"=w521, "Num Event Frames"=w526) -> ("Event Frame?"=w525:bool)  [unwired: 7 in, 1 out]
            n175 = Index Array(array=w531, index=w521) -> (element=w528:string)
            n176 = Not(x=w542) -> (.not. x?=w541:bool)
            n177 = call "Display Message to User"("Enable"=w541) -> ()  [unwired: 9 in, 2 out]
            n178 = Decrement(x=w521) -> (x-1=w520:i32)
            n179 = call "Set Visible State.vi"("Event Structure Frame (-1: Use State Name)"=w520, "Event Structure (F: Case Structure)"=w525, "error in (no error)"=w523, "State Name"=w528, "JKI SM in"=w529) -> ("error out"=w527:errorcluster)  [unwired: 5 in, 1 out]
            n180 = Bundle By Name(cluster=w548, "NavIndex"=w540, "SelectedCase"=w550, "tag"=w528) -> (w549:T13)
            n181 = call <vilib>:"Add State(s) to Queue__jki_lib_state_machine.vi"("State(s) in Front (\"\")"="UI: Update" ("State(s) in Front (\"\")"), "State(s) in (\"\")"=w536) -> ("States Out"=w535:string)  [unwired: 13 in]
          }
          event Value Change {
            n182 = event-data() -> ()  [unwired: 7 out]
            n183 = call <vilib>:"Add State(s) to Queue__jki_lib_state_machine.vi"("State(s) in Front (\"\")"="Navigation: Clear History\nUI: Update" ("State(s) in Front (\"\")"), "State(s) in (\"\")"=w555) -> ("States Out"=w554:string)  [unwired: 13 in]
          }
          event Value Change {
            n184 = event-data() -> ()  [unwired: 7 out]
            n185 = call <vilib>:"Add State(s) to Queue__jki_lib_state_machine.vi"("State(s) in Front (\"\")"="Macro: update list" ("State(s) in Front (\"\")"), "State(s) in (\"\")"=w559) -> ("States Out"=w560:string)  [unwired: 13 in]
          }
          event "Add macro": Value Change {
            n186 = event-data() -> ()  [unwired: 2 out]
          }
          event Panel Close? {
            # "Discard the event because we'll close the front panel ourselves in Macro: Exit"
            # "Close Panel button (pressed) Event\n(this executes Macro: Exit to terminate the VI)"
            n187 = event-data() -> ()  [unwired: 2 out]
            n188 = event-data("Discard?"=TRUE) -> ()  [unwired: 1 in, 1 out]
            n189 = call <vilib>:"Add State(s) to Queue__jki_lib_state_machine.vi"("State(s) in Front (\"\")"="Macro: Exit", "State(s) in (\"\")"=w573) -> ("States Out"=w572:string)  [unwired: 1 in, 12 out]
          }
        }
      }
      frame "---------- Core ----------" {
        # "Do not put any code in this frame.\n(it is a separator no-op)"
      }
      frame Default {
        w585 = 42 items=["No error", "Argument error", "Memory is full", "Out of zone", "End of file", "File already open", "Generic file I/O error", "File not found", "File permission error", "Disk is full", "Duplicate path", "Too many files open", "System feature not enabled", "Resource file not found", "Cannot add resource", "Resource not found", "Image not found", "Image memory error", "Pen does not exist", "Config type invalid", "Config token not found", "Config parse error", "Config memory error", "Bad external code format", "Bad external code offset", "External code not present", "Null window", "Destroy window error", "Null menu", "Print aborted", "Bad print record", "Print driver error", "Windows error during printing", "Memory error during printing", "Print dialog error", "Generic print error", "Invalid device refnum", "Device not found", "Device parameter error", "Device unit error", "Cannot open device", "Device call aborted", "Generic error", "Cancelled by user", "Object ID too low", "Object ID too high", "Object not in heap", "Unknown heap", "Unknown object (invalid DefProc)", "Unknown object (DefProc not in table)", "Message out of range", "Invalid (null) method", "Unknown message", "Manager call not supported", "Bad address", "Network operation in progress", "Network operation timed out", "Connection is busy", "Network attribute not supported", "Network error", "Address in use", "System out of memory", "Connection aborted", "Connection refused", "Not connected", "Already connected", "Connection closed", "Initialization error (interapplication manager)", "Bad occurrence", "Wait on unbound occurrence handler", "Occurrence queue overflow", "Datalog type conflict", "Unused", "Unrecognized type (interapplication manager)", "Memory corrupt", "Failed to make temporary DLL", "Old CIN version", "Drag socket not found", "Failed to load drop-object", "Failed to register OLE object", "Failed to release OLE object", "Format specifier type mismatch", "Unknown format specifier", "Too few format specifiers", "Too many format specifiers", "Scan failed", "Newer CIN version", "Error converting to variant", "Runtime menu error", "Password tampered", "Variant attribute not found", "Incompatible variant data type", "Event data is not available", "Event Store is not present", "Occurrence is not found", "Event Queue is not created", "Event info is not available", "Refnum passed is NULL", "Error retrieving Class GUID", "Error retrieving CoClass GUID", "Error retrieving TypeLib GUID.", "Bad built application magic bytes.", "Specific driver is different from the specific driver associated with the Logical Name.", "There is no session opened to the class driver.", "Max Error", "MAX - Error with config objects", "MAX - Error loading configuration", "MAX - Group not supported"]
        # "Current State"
        # "Do not delete, rename, or modify this frame.\n(this is used to capture unhandled states and typos)"
        # "Handle mistyped state name (developer tool)"
        n190 = Format Into String(format string="Software Exception: Unhandled State \"%s\"." ("message"), error in=w581, w578) -> (resulting string=w584:string, error out=w583:errorcluster)  [unwired: 1 in]
        n191 = call <vilib>:"Error Cluster From Error Code.vi"("show call chain? (False)"=TRUE, "error in (no error)"=w583, "error message (\"\")"=w584, "error code (0)"=w585) -> ("error out"=w582:errorcluster)  [unwired: 5 out]
      }
      frame "Initialize Core Data" {
        # "Do not delete, rename, or modify this frame.\n(this is used to determine panel behavior on exit)"
        # "originally closed?"
        # "exe?"
        # "If panel starts closed or is an EXE, then close it when we exit"
        n192 = property class="VI"() -> ("Front Panel.Open"=w595:bool)  [unwired: 2 in, 2 out]
        n193 = property class="App"() -> ("App.Kind"=w594:T8)  [unwired: 2 in, 2 out]
        n194 = control-ref of="Current VI Reference"() -> (w588:refnum<vi>)
        n195 = Not(x=w595) -> (.not. x?=w592:bool)
        n196 = Equal?(x=w594, y=T8."Run Time System" ("Application:Kind")) -> (x = y?=w591:bool)
        n197 = Or(x=w592, y=w591) -> (x .or. y?=w589:bool)
        n198 = Bundle By Name(cluster=w590, "Core.Current VI Reference"=w588, "Core.Close Panel on Exit?"=w589) -> (w597:T13)
      }
      frame "Mass Compile Self" {
        w602 = FALSE  # Allow self mass compile
        # "Installed beneath LabVIEW?"
        # "child path?"
        # "Do not delete, rename, or modify this frame.\n(this is used to determine panel behavior on exit)"
        n199 = call <vilib>:"Application Directory.vi"() -> ("Application Directory"=w605:path)
        n200 = call-poly <userlib>:"Build Path__ogtk.vi"("name or relative path"=path[] [path "resource/dialog/QuickDrop/plugins/JKI State Machine Helper__JKI_State_Machine_Helper.vi", path "resource/plugins/PopupMenus/edit time panel and diagram/JKI SM Helper.llb", path "resource/dialog/QuickDrop/plugins/JKI State Machine API", path "resource/dialog/QuickDrop/plugins/_JKI State Machine Helper"], "base path"=w605) -> ("appended path"=w603:path[])
        n201 = call <vilib>:"Application Directory.vi"() -> ("Application Directory"=w600:path)
        n202 = Current VI's Path() -> (path=w599:path)
        n203 = call "Is Child Path -- JKI State Machine Editor.vi"("Path"=w599, "Parent Directory"=w600) -> ("is Child Path?"=w598:bool)
        n204 = Or(x=w602, y=w598) -> (x .or. y?=w601:bool)
        n205 = case shown="True" w601 {
          tunnel: w603 -> [_ w609]
          frame False {
          }
          frame True {
            n206 = call "Mass Compile LabVIEW Tool.vi"("Product Folders"=w609, "Product Name"="JKI State Machine Editor") -> ()  [unwired: 8 in, 2 out]
          }
        }
      }
      frame "Error Handler" {
        w631 = i32[] [1055, 1026]  # Errors signaling shutdown (invalid references, etc.)
        # "This is is to avoid getting into shutdown loops.\nIf there was an error during init, then the refs aren't valid, so that causes more errors, and we get back here."
        # "Clear Errors"
        # "Clear Errors if Known Error Signaling a Need to Shutdown"
        # "Error Dialog"
        # "Handle any errors here.\nYou can also output any states to clean-up after errors occur"
        n207 = call <vilib>:"Append Error Details__jki_lib_state_machine.vi"("error in (no error)"=w619, "Previous State and Argument(s)"=w617) -> ("error out"=w618:errorcluster)  [unwired: 9 in]
        n208 = Unbundle By Name(w618) -> ("code"=w629:i32)
        n209 = Unbundle By Name(w624) -> ("Error During Startup"=w623:bool)
        n210 = Search 1D Array(1D array=w631, element=w629) -> (index of element=w630:i32)  [unwired: 1 out]
        n211 = Greater Or Equal To 0?(x=w630) -> (x >= 0?=w615:bool)
        n212 = call <vilib>:"Clear Errors.vi"("error in (no error)"=w618) -> ("error out"=w628:errorcluster)  [unwired: 1 in, 5 out]
        n213 = Select(t=w628, s=w615, f=w618) -> (s? t:f=w627:errorcluster)
        n214 = Unbundle By Name(w624) -> ("Undo Transaction"=w612:bool)
        n215 = call <vilib>:"Simple Error Handler.vi"("error in (no error)"=w627) -> ("error out"=w626:errorcluster)  [unwired: 4 in, 4 out]
        n216 = call <vilib>:"Clear Errors.vi"("error in (no error)"=w626) -> ("error out"=w625:errorcluster)  [unwired: 1 in, 5 out]
        n217 = call <vilib>:"Conditional State String__jki_lib_state_machine.vi"("Do State(s)?"=w615, "State"="Macro: Exit" ("t")) -> ("State Out"=w614:string)  [unwired: 7 in]
        n218 = call <vilib>:"Conditional State String__jki_lib_state_machine.vi"("Do State(s)?"=w612, "State"="Script: fail undo") -> ("State Out"=w611:string)  [unwired: 7 in]
        n219 = call <vilib>:"Add State(s) to Queue__jki_lib_state_machine.vi"("State(s) in Front (\"\")"=w614, "State(s) at Back (\"\")"=w611) -> ("States Out"=w622:string)  [unwired: 1 in, 12 out]
        n220 = call-poly <vilib>:"Select State(s)__jki_lib_state_machine.vi"("State(s) if True (\"\")"="Exit" ("t"), "Select"=w623, "State(s) if False (\"\")"=w622) -> ("States Out"=w621:string)  [unwired: 12 in]
      }
      frame "Exit" {
        # "Do not put any code in this frame.\n(No errors that occur here will be handled.)"
      }
      frame "---------- Data ----------" {
        # "Do not put any code in this frame.\n(It is a separator no-op. You can make a copy of this frame to create a new Data frame)"
      }
      frame "Data: Initialize" {
        w645 = refnum<vi>[] []  # OpenCategoryFrames
        w646 = refnum<vi>[] []  # Frames[]
        w647 = 0  # Num Event Frames
        w653 = refnum<class "JKI SM.lvclass"> refnum  # JKI SM
        w654 = -1  # Top Row Index
        w655 = TRUE  # Undo Transaction
        w660 = -1  # NavIndex
        w661 = refnum<vi>[] []  # NavHist
        w664 = ""  # TempString
        w666 = ""  # CaseStrVIName
        w667 = ""  # SectHdr
        w668 = "----------"  # TreeSectHdrs
        w673 = T12 {"Left"=0, "Top"=0, "Right"=0, "Bottom"=0}  # Display:Primary Workspace
        w675 = ""  # Top Row Tag
        w676 = ""  # tag
        w677 = u32 0  # SelectedCase
        w680 = 0  # DisplayedItems
        w681 = string[] []  # FrameNames
        w684 = T14 {"Current VI Reference"=refnum, "Close Panel on Exit?"=FALSE}  # Core
        w663 = FALSE  # Ctrl?
        w665 = FALSE  # Activating
        w674 = refnum<vi> refnum  # CaseStrVI Ref
        w662 = refnum<vi> refnum  # StructRef
        w682 = FALSE  # InBounds
        w683 = FALSE  # Indent?
        # "screen size"
        n221 = control-ref of="Tree"() -> (w678:refnum<vi>)
        n222 = call "Create (From GObject).vi"("error in (no error)"=w651, "GObject"=w640) -> ("error out"=w650:errorcluster, "JKI SM out"=w644:refnum<class "JKI SM.lvclass">)  [unwired: 6 in, 2 out]
        n223 = call "Check Is Helper Already Running (Get Queue) -- Wrapper.vi"("Create? (F: Check)"=TRUE, "JKI SM in"=w644) -> ()  [unwired: 8 in, 2 out]
        n224 = call "Get VI Reference.vi"("error in (no error)"=w650, "JKI SM in"=w644) -> ("error out"=w648:errorcluster, "JKI SM out"=w649:refnum<class "JKI SM.lvclass">)  [unwired: 7 in, 1 out]
        n225 = Open Application Reference(8:w648) -> (0:w671:errorcluster, 3:w672:refnum<vi>)  [unwired: 3 in]
        n226 = Variant To Data(type=w653, Variant=w649) -> (data=w652:refnum<class "JKI SM.lvclass">)  [unwired: 1 in, 1 out]
        n227 = property class="App"(reference=w672, error in=w671) -> (error out=w670:errorcluster, "Disp.WkSpace"=w669:T12)  [unwired: 1 out]
        n228 = Close Reference(reference=w672, error in (no error)=w670) -> (error out=w658:errorcluster)
        n229 = property class="VI"(reference=w639) -> ("Name"=w659:string)  [unwired: 1 in, 2 out]
        n230 = property class="VI"(error in=w658, "Front Panel.Title"=w659) -> (error out=w643:errorcluster)  [unwired: 1 in, 1 out]
        n231 = call "ErrorDuringStartup.vi"("error in"=w643) -> ("error out"=w641:errorcluster, "Error During Startup"=w642:bool)  [unwired: 9 in]
        n232 = Bundle("OpenCategoryFrames"=w645, "Frames[]"=w646, "Core"=w684, "Indent?"=w683, "InBounds"=w682, "Activating"=w665, "FrameNames"=w681, "tag"=w676, "Top Row Tag"=w675, "TreeSectHdrs"=w668, "SectHdr"=w667, "CaseStrVIName"=w666, "TempString"=w664, "DisplayedItems"=w680, "SelectedCase"=w677, "Display:Primary Workspace"=w673, "Tree"=w678, "StructRef"=w662, "CaseStrVI Ref"=w674, "Ctrl?"=w663, "NavHist"=w661, "NavIndex"=w660, "Undo Transaction"=w655, "Top Row Index"=w654, "JKI SM"=w652, "Num Event Frames"=w647, "Error During Startup"=w642) -> (w685:T13)  [unwired: 1 out]
        n233 = Bundle By Name(cluster=w685, "CaseStrVIName"=w659, "CaseStrVI Ref"=w639, "Display:Primary Workspace"=w669) -> (w679:T13)
      }
      frame "Data: get section header" {
        w691 = TRUE ("replace all? (F)")
        n234 = Unbundle By Name(w697) -> ("TreeSectHdrs"=w687:string, "FrameNames"=w686:string[], "tag"=w689:string)
        n235 = while {
          tunnel: w686 -> [w701] mode=indexing
          tunnel: w689 -> [w707]
          tunnel: w687 -> [w704]
          shift-right: [w703] -> w693
          shift-left: "" -> [w702]
          stop <- w700 stop-if-true
          n236 = Equal?(x=w701, y=w707) -> (x = y?=w700:bool)
          n237 = Match Pattern(string=w701, regular expression=w704) -> (offset past match=w706:i32)  [unwired: 4 out]
          n238 = Less Than 0?(x=w706) -> (x < 0?=w705:bool)
          n239 = Select(t=w702, s=w705, f=w701) -> (s? t:f=w703:string)
        }
        n240 = Search and Replace String(replace all?=w691, input string=w693, search string="\"") -> (result string=w692:string)  [unwired: 1 in, 7 out]
        n241 = Search and Replace String(replace all?=w691, input string=w692, search string=w687) -> (result string=w694:string)  [unwired: 1 in, 7 out]
        n242 = call <vilib>:"Trim Whitespace.vi"("string"=w694) -> ("trimmed string"=w688:string)  [unwired: 1 in]
        n243 = Bundle By Name(cluster=w697, "SectHdr"=w688) -> (w696:T13)
      }
      frame "Data: get drop section hdr" {
        # "Get the index of the frame before"
        n244 = Unbundle By Name(w713) -> ("FrameNames"=w711:string[])
        n245 = property on="Tree" class="Tree (strict)"() -> ("All Tags"=w712:string[])  [unwired: 2 in, 2 out]
        n246 = while {
          tunnel: w711 -> [w717]
          tunnel: w712 -> [w716] mode=indexing
          tunnel: [w718] -> w710
          i -> [w719]
          stop <- w720 stop-if-true
          n247 = call "Search for Frame in Frames.vi"("Frame Name"=w716, "Frame Names"=w717) -> ("index of element"=w721:i32)  [unwired: 9 in]
          n248 = Decrement(x=w719) -> (x-1=w718:i32)
          n249 = Less Than 0?(x=w721) -> (x < 0?=w720:bool)
        }
        n250 = Index Array(array=w711, index=w710) -> (element=w708:string)
        n251 = Bundle By Name(cluster=w713, "tag"=w708) -> (w709:T13)
      }
      frame "Data: Cleanup" {
        # "Ignore Errors at Shutdown"
        # "Cleanup any data and references, here.\n(this is called automatically, by the Macro: Exit)"
        n252 = Unbundle By Name(w729) -> ("JKI SM"=w726:refnum<class "JKI SM.lvclass">, "Core.Current VI Reference"=w730:refnum<vi>)
        n253 = Close Reference(reference=w730, error in (no error)=w727) -> (error out=w723:errorcluster)
        n254 = call "Destroy.vi"("error in (no error)"=w723, "JKI SM in"=w726) -> ("error out"=w725:errorcluster)  [unwired: 9 in]
        n255 = call <vilib>:"Clear Errors.vi"("error in (no error)"=w725) -> ("error out"=w724:errorcluster)  [unwired: 5 in, 1 out]
        n256 = Merge Errors(w723, w724) -> (w722:errorcluster)
      }
      frame "---------- UI ----------" {
        # "Do not put any code in this frame.\n(It is a separator no-op. You can make a copy of this frame to create a new UI frame)"
      }
      frame "UI: Initialize" {
        w737 = T15."Disabled and Grayed Out" ("Disabled")
        # "Initialize the User Interface, here.\n(this is called automatically, by the Macro: Init)"
        n257 = property on="Back" class="Bool"("DisabledEnum"=w737) -> ()  [unwired: 2 in, 2 out]
        n258 = property on="Forward" class="Bool"("DisabledEnum"=w737) -> ()  [unwired: 2 in, 2 out]
        n259 = property on="Clear History" class="Bool"("DisabledEnum"=w737) -> ()  [unwired: 2 in, 2 out]
        n260 = property on="Search Icon" class="Bool (strict)"("Visible"=TRUE) -> ()  [unwired: 2 in, 2 out]
        n261 = property on="Clear Search" class="Bool (strict)"("Visible"=FALSE) -> ()  [unwired: 2 in, 2 out]
        n262 = local write "Search"("") -> ()
      }
      frame "UI: Update" {
        w748 = T15."Enabled" ("Disabled")
        w749 = T15."Disabled and Grayed Out" ("Disabled")
        # "Initialize the User Interface, here.\n(this is called automatically, by the Macro: Init)"
        n263 = Unbundle By Name(w753) -> ("NavIndex"=w747:i32, "NavHist"=w745:refnum<vi>[])
        n264 = Array Size(array=w745) -> (size(s)=w746:i32)
        n265 = Increment(x=w747) -> (x+1=w744:i32)
        n266 = Less Or Equal To 0?(x=w747) -> (x <= 0?=w741:bool)
        n267 = Equal?(x=w746, y=w744) -> (x = y?=w743:bool)
        n268 = Empty Array?(array=w745) -> (empty?=w752:bool)
        n269 = Select(t=w749, s=w752, f=w748) -> (s? t:f=w751:T15)
        n270 = Select(t=w749, s=w741, f=w748) -> (s? t:f=w750:T15)
        n271 = Select(t=w749, s=w743, f=w748) -> (s? t:f=w742:T15)
        n272 = property on="Back" class="Bool"("DisabledEnum"=w750) -> ()  [unwired: 2 in, 2 out]
        n273 = property on="Forward" class="Bool"("DisabledEnum"=w742) -> ()  [unwired: 2 in, 2 out]
        n274 = property on="Clear History" class="Bool"("DisabledEnum"=w751) -> ()  [unwired: 2 in, 2 out]
      }
      frame "UI: Front Panel State" {
        # "Set Front Panel Open or Closed\n(Usage: \"UI: Front Panel State >> Open|Close\")"
        n275 = Unbundle By Name(w759) -> ("Core.Current VI Reference"=w758:refnum<vi>)
        n276 = case shown="\"Open\", Default" w756 {
          tunnel: w761 -> [w765 w778]
          tunnel: [w767 w779] -> w760
          tunnel: w758 -> [w766 w776]
          frame "Open", Default {
            n277 = property class="VI"(reference=w766, error in=w765) -> (reference out=w763:refnum<vi>, error out=w764:errorcluster, "Front Panel.Open"=w762:bool)
            n278 = case shown="False" w762 {
              tunnel: [w770 w773] -> w767
              tunnel: w764 -> [w769 w773]
              tunnel: w763 -> [w768 _]
              frame False {
                n279 = invoke class="VI" method="FP.Open"(reference=w768, error in=w769, "Activate"=TRUE, "State"=T6."Standard") -> (error out=w770:errorcluster)  [unwired: 1 in, 4 out]
              }
              frame True {
              }
            }
          }
          frame "Close" {
            n280 = property class="VI"(reference=w776, error in=w778) -> (reference out=w775:refnum<vi>, error out=w777:errorcluster, "Front Panel.Open"=w774:bool)
            n281 = case shown="True" w774 {
              tunnel: [w780 w783] -> w779
              tunnel: w777 -> [w780 w782]
              tunnel: w775 -> [_ w781]
              frame False {
              }
              frame True {
                n282 = invoke class="VI" method="FP.Close"(reference=w781, error in=w782) -> (error out=w783:errorcluster)  [unwired: 1 in, 2 out]
              }
            }
          }
        }
      }
      frame "UI: front panel size" {
        # "FP width"
        # "reposition panel"
        # "top = screen bottom - panel height"
        # "left = screen right - panel width"
        # "panel size"
        n283 = Unbundle By Name(w798) -> ("Display:Primary Workspace.Right"=w788:i16, "Display:Primary Workspace.Bottom"=w787:i16, "Core.Current VI Reference"=w789:refnum<vi>)  [unwired: 2 out]
        n284 = property class="VI"(reference=w789, error in=w797) -> (reference out=w785:refnum<vi>, error out=w786:errorcluster, "Front Panel.WinBounds"=w793:T12)
        n285 = Unbundle By Name(w793) -> ("Right"=w794:i16, "Left"=w795:i16)
        n286 = Subtract(x=w794, y=w795) -> (x-y=w790:i16)
        n287 = Subtract(x=w788, y=w790) -> (x-y=w791:i16)
        n288 = Bundle By Name(cluster=w793, "Right"=w788, "Bottom"=w787, "Left"=w791, "Top"=i16 0 ("x-y")) -> (w792:T12)
        n289 = property class="VI"(reference=w785, error in=w786, "Front Panel.WinBounds"=w792) -> (error out=w796:errorcluster)  [unwired: 1 out]
      }
      frame "UI: defer panel updates" {
        n290 = Unbundle By Name(w814) -> ("Core.Current VI Reference"=w813:refnum<vi>)
        n291 = call <vilib>:"Trim Whitespace.vi"("string"=w812) -> ("trimmed string"=w811:string)  [unwired: 1 in]
        n292 = Equal?(x=w811, y="TRUE") -> (x = y?=w800:bool)
        n293 = property class="VI"(reference=w813, error in=w816) -> (error out=w804:errorcluster, "Panel"=w806:refnum<vi>)  [unwired: 1 out]
        n294 = property class="Pnl"(reference=w806, error in=w804) -> (reference out=w805:refnum<vi>, error out=w803:errorcluster, "DeferPanUpdts"=w802:bool)
        n295 = Not Equal?(x=w800, y=w802) -> (x != y?=w801:bool)
        n296 = case "Requested Value is Different than Current Value? Then: Set Property" shown="True" w801 {
          tunnel: [w817 w822] -> w815
          tunnel: [_ w821] -> w807
          tunnel: w805 -> [_ w820]
          tunnel: w803 -> [w817 w819]
          tunnel: w800 -> [_ w818]
          frame False {
            # "No Op"
          }
          frame True {
            n297 = property class="Pnl"(reference=w820, error in=w819, "DeferPanUpdts"=w818) -> (error out=w822:errorcluster)  [unwired: 1 out]
            n298 = case shown="True" w818 {
              tunnel: [_ "UI: defer panel updates >> FALSE" ("State(s) at Back (\"\")")] -> w821
              frame False {
              }
              frame True {
                # "Un-defer updates *after* all states finish"
              }
            }
          }
        }
        n299 = call <vilib>:"Add State(s) to Queue__jki_lib_state_machine.vi"("State(s) in (\"\")"=w809, "State(s) at Back (\"\")"=w807) -> ("States Out"=w808:string)  [unwired: 1 in, 12 out]
      }
      frame "UI: show/hide scroll bar" {
        n300 = Unbundle By Name(w831) -> ("FrameNames"=w829:string[], "Tree"=w830:refnum<vi>)
        n301 = call "ShowHideScrollBar.vi"("error in"=w833, "reference"=w830) -> ("error out"=w832:errorcluster, "Visible?"=w824:bool)  [unwired: 8 out]
        n302 = case shown="False" w824 {
          tunnel: w831 -> [w839 w840]
          tunnel: w829 -> [w838 _]
          tunnel: [w837 w840] -> w828
          tunnel: ["UI: restore position" _] -> w825
          frame False {
            w834 = 0 ("Top Row Index")
            # "Set the position to the top\nif the scroll bar isn't visible."
            n303 = Index Array(array=w838, index=w834) -> (element=w836:string)
            n304 = Bundle By Name(cluster=w839, "Top Row Tag"=w836, "Top Row Index"=w834) -> (w837:T13)
          }
          frame True {
          }
        }
        n305 = call <vilib>:"Add State(s) to Queue__jki_lib_state_machine.vi"("State(s) in Front (\"\")"=w825, "State(s) in (\"\")"=w827) -> ("States Out"=w826:string)  [unwired: 1 in, 12 out]
      }
      frame "UI: collapse/expand tree" {
        n306 = Unbundle By Name(w850) -> ("Frames[]"=w841:refnum<vi>[], "FrameNames"=w843:string[], "Tree"=w842:refnum<vi>)
        n307 = Equal?(x=w854, y="Expand All") -> (x = y?=w847:bool)
        n308 = invoke class="Tree (strict)" method="Open/Close.Open/Close All"(reference=w842, error in=w855, "Open"=w847) -> (reference out=w846:refnum<vi>, error out=w845:errorcluster)  [unwired: 1 in, 2 out]
        n309 = Index Array(array=w843) -> (element=w848:string)  [unwired: 1 in]
        n310 = case shown="False" w847 {
          tunnel: w845 -> [w866 w870]
          tunnel: [w865 w870] -> w856
          tunnel: w846 -> [w864 _]
          tunnel: w848 -> [w861 _]
          tunnel: w850 -> [w859 w869]
          tunnel: w841 -> [_ w868]
          tunnel: [w858 w867] -> w849
          frame False {
            # "Put the first case at\nthe top of the Tree\nso it doesn't collapse\nand hide the stuff\nat the top of the list."
            n311 = Bundle By Name(cluster=cluster{"Node":string, "Column":i32} {"Node"="", "Column"=0} ("Top Left Visible Cell"), "Node"=w861, "Column"=0) -> (w862:cluster{"Node":string, "Column":i32})
            n312 = Bundle By Name(cluster=w859, "OpenCategoryFrames"=refnum<vi>[] [] ("FrameIsOpen")) -> (w858:T13)
            n313 = property class="Tree (strict)"(reference=w864, error in=w866, "TopLeft"=w862) -> (error out=w865:errorcluster)  [unwired: 1 out]
          }
          frame True {
            n314 = Bundle By Name(cluster=w869, "OpenCategoryFrames"=w868) -> (w867:T13)
          }
        }
        n315 = call <vilib>:"Add State(s) to Queue__jki_lib_state_machine.vi"("State(s) in Front (\"\")"="UI: show/hide scroll bar", "State(s) in (\"\")"=w852) -> ("States Out"=w851:string)  [unwired: 1 in, 12 out]
      }
      frame "UI: restore position" {
        n316 = Unbundle By Name(w880) -> ("Top Row Index"=w875:i32, "Tree"=w871:refnum<vi>)
        n317 = property class="Tree (strict)"(reference=w871, error in=w882) -> (reference out=w872:refnum<vi>, error out=w873:errorcluster, "DispItems"=w876:string[])
        n318 = Index Array(array=w876, index=w875) -> (element=w874:string)
        n319 = Empty String/Path?(string/path=w874) -> (empty?=w878:bool)
        n320 = Not(x=w878) -> (.not. x?=w877:bool)
        n321 = case shown="True" w877 {
          tunnel: w873 -> [w883 w890]
          tunnel: [w883 w889] -> w879
          tunnel: w874 -> [_ w885]
          tunnel: w872 -> [_ w884]
          frame False {
          }
          frame True {
            n322 = Bundle By Name(cluster=cluster{"Node":string, "Column":i32} {"Node"="", "Column"=0} ("Top Left Visible Cell"), "Node"=w885, "Column"=0) -> (w886:cluster{"Node":string, "Column":i32})
            n323 = property class="Tree (strict)"(reference=w884, error in=w890, "TopLeft"=w886) -> (error out=w889:errorcluster)  [unwired: 1 out]
          }
        }
      }
      frame "UI: select message" {
        n324 = One Button Dialog(message="Nothing is selected.") -> ()  [unwired: 2 out]
      }
      frame "---------- Macro ----------" {
        # "Do not put any code in this frame.\n(It is a separator no-op. You can make a copy of this frame to create a new Macro frame)"
      }
      frame "Macro: Initialize" {
        w898 = "Data: Initialize\nInitialize Core Data\nUI: Initialize\n\n//Script: get CaseStruct Ref\nMacro: process structure\nUI: collapse/expand tree >> Expand All\n\nUI: Update\nUI: show/hide scroll bar\nUI: front panel size\nUI: Front Panel State >> Open"  # Data: Initialize Initialize Core Data UI: Initialize  //Script: get CaseStruct Ref Macro: process structure UI: collapse/expand tree >> Expand All  UI: Update UI: show/hide scroll bar UI: front panel size UI: Front Panel State >> Open
        # "Initialization Macro\n(This is called once, when the VI starts)"
        n325 = call <vilib>:"Add State(s) to Queue__jki_lib_state_machine.vi"("State(s) in Front (\"\")"=w898, "State(s) in (\"\")"=w902) -> ("States Out"=w901:string)  [unwired: 1 in, 12 out]
      }
      frame "Macro: process structure" {
        n326 = call <vilib>:"Add State(s) to Queue__jki_lib_state_machine.vi"("State(s) in Front (\"\")"=w903, "State(s) in (\"\")"=w905) -> ("States Out"=w904:string)  [unwired: 13 in]
      }
      frame "Macro: insert" {
        n327 = Search and Replace String(input string="Data: get section header\nScript: begin undo >> insert\nScript: insert frame >> [FRAME]\nScript: Mark calling VI Modified\nScript: end undo", search string="[FRAME]", replace string=w908) -> (result string=w910:string)  [unwired: 5 in, 3 out]
        n328 = call <vilib>:"Add State(s) to Queue__jki_lib_state_machine.vi"("State(s) in Front (\"\")"=w910, "State(s) in (\"\")"=w913) -> ("States Out"=w912:string)  [unwired: 1 in, 12 out]
      }
      frame "Macro: delete" {
        n329 = Search and Replace String(input string=w916, search string="[FRAME]", replace string=w919, error in=w918) -> (result string=w920:string, error out=w917:errorcluster)  [unwired: 4 in, 2 out]
        n330 = call <vilib>:"Add State(s) to Queue__jki_lib_state_machine.vi"("State(s) in Front (\"\")"=w920, "State(s) in (\"\")"=w923) -> ("States Out"=w922:string)  [unwired: 13 in]
      }
      frame "Macro: Select Case" {
        # "Visible frame not the indext we think it should be?"
        n331 = Unbundle By Name(w935) -> ("tag"=w928:string, "JKI SM"=w932:refnum<class "JKI SM.lvclass">)
        n332 = call "Get All Case and Event Frames.vi"("error in (no error)"=w933, "JKI SM in"=w932) -> ("error out"=w930:errorcluster, "Frame Names"=w931:string[], "Visible Frame Index"=w929:i32)  [unwired: 1 in, 6 out]
        n333 = call "Search for Frame in Frames.vi"("Frame Name"=w928, "Frame Names"=w931) -> ("index of element"=w936:i32)  [unwired: 9 in]
        n334 = To Unsigned Long Integer(number=w936) -> (unsigned 32bit integer=w934:u32)
        n335 = Not Equal?(x=w934, y=w929) -> (x != y?=w926:bool)
        n336 = Search and Replace String(input string="Script: begin undo >> Visible Frame Changed\nScript: select case\nScript: end undo\n//Script: do undo", search string="[FRAME]", replace string=w938, error in=w930) -> (result string=w927:string, error out=w937:errorcluster)  [unwired: 4 in, 2 out]
        n337 = call <vilib>:"Conditional State String__jki_lib_state_machine.vi"("Do State(s)?"=w926, "State"=w927) -> ("State Out"=w925:string)  [unwired: 7 in]
        n338 = call <vilib>:"Add State(s) to Queue__jki_lib_state_machine.vi"("State(s) in Front (\"\")"=w925, "State(s) in (\"\")"=w942) -> ("States Out"=w941:string)  [unwired: 13 in]
      }
      frame "Macro: update list" {
        n339 = call <vilib>:"Add State(s) to Queue__jki_lib_state_machine.vi"("State(s) in Front (\"\")"=w943, "State(s) in (\"\")"=w945) -> ("States Out"=w944:string)  [unwired: 1 in, 12 out]
      }
      frame "Macro: process drag-copy" {
        n340 = call <vilib>:"Add State(s) to Queue__jki_lib_state_machine.vi"("State(s) in Front (\"\")"="Data: get drop section hdr\nData: get section header\nScript: process drag-copy\nScript: select case\nScript: Mark calling VI Modified" ("message"), "State(s) in (\"\")"=w951) -> ("States Out"=w950:string)  [unwired: 1 in, 12 out]
      }
      frame "Macro: sort list" {
        n341 = call <vilib>:"Add State(s) to Queue__jki_lib_state_machine.vi"("State(s) in Front (\"\")"="Script: begin undo >> sort\nScript: sort list\nScript: end undo\nMacro: update list\nUI: collapse/expand tree >> Expand All", "State(s) in (\"\")"=w955) -> ("States Out"=w954:string)  [unwired: 1 in, 12 out]
      }
      frame "Macro: rename" {
        n342 = Search and Replace String(input string=w958, search string="[FRAME]", replace string=w959, error in=w963) -> (result string=w961:string, error out=w962:errorcluster)  [unwired: 4 in, 2 out]
        n343 = call <vilib>:"Add State(s) to Queue__jki_lib_state_machine.vi"("State(s) in Front (\"\")"=w961, "State(s) in (\"\")"=w966) -> ("States Out"=w965:string)  [unwired: 1 in, 12 out]
      }
      frame "Macro: duplicate" {
        n344 = Search and Replace String(input string="Data: get section header\nScript: begin undo >> rename\nScript: duplicate case >> [FRAME]\nScript: Mark calling VI Modified\nScript: end undo\nMacro: update list", search string="[FRAME]", replace string=w971, error in=w970) -> (result string=w967:string, error out=w969:errorcluster)  [unwired: 4 in, 2 out]
        n345 = call <vilib>:"Add State(s) to Queue__jki_lib_state_machine.vi"("State(s) in Front (\"\")"=w967, "State(s) in (\"\")"=w974) -> ("States Out"=w973:string)  [unwired: 1 in, 12 out]
      }
      frame "Macro: Add Dynamic Events" {
        n346 = call <vilib>:"Add State(s) to Queue__jki_lib_state_machine.vi"("State(s) in Front (\"\")"=w976, "State(s) in (\"\")"=w979) -> ("States Out"=w978:string)  [unwired: 1 in, 12 out]
      }
      frame "Macro: Find Callers" {
        n347 = Search and Replace String(input string="Script: Find Callers >> [FRAME]", search string="[FRAME]", replace string=w985, error in=w984) -> (result string=w981:string, error out=w983:errorcluster)  [unwired: 4 in, 2 out]
        n348 = call <vilib>:"Add State(s) to Queue__jki_lib_state_machine.vi"("State(s) in Front (\"\")"=w981, "State(s) in (\"\")"=w988) -> ("States Out"=w987:string)  [unwired: 1 in, 12 out]
      }
      frame "Macro: drop state name" {
        n349 = call <vilib>:"Add State(s) to Queue__jki_lib_state_machine.vi"("State(s) in Front (\"\")"="Script: begin undo >> drop\nScript: drop state name\nScript: Mark calling VI Modified\nScript: end undo" ("t"), "State(s) in (\"\")"=w992) -> ("States Out"=w991:string)  [unwired: 13 in]
      }
      frame "Macro: append string" {
        n350 = call <vilib>:"Add State(s) to Queue__jki_lib_state_machine.vi"("State(s) in Front (\"\")"="Script: begin undo >> append\nScript: append string\nScript: Mark calling VI Modified\nScript: end undo" ("t"), "State(s) in (\"\")"=w997) -> ("States Out"=w996:string)  [unwired: 13 in]
      }
      frame "Macro: copy frame" {
        n351 = Match Pattern(string=w1004, regular expression=",") -> (before substring=w1002:string, after substring=w1001:string)  [unwired: 1 in, 2 out]
        n352 = Format Into String(format string="Script: begin undo >> copy\nScript: copy frame >> %s,%s\nScript: Mark calling VI Modified\nScript: end undo", w1002, w1001) -> (resulting string=w1000:string)  [unwired: 2 in, 1 out]
        n353 = call <vilib>:"Add State(s) to Queue__jki_lib_state_machine.vi"("State(s) in Front (\"\")"=w1000, "State(s) in (\"\")"=w1007) -> ("States Out"=w1006:string)  [unwired: 13 in]
      }
      frame "Macro: Exit" {
        # "Exit Macro\n(This is called once, when the VI exits)"
        n354 = call <vilib>:"Add State(s) to Queue__jki_lib_state_machine.vi"("State(s) in Front (\"\")"="UI: Front Panel State >> Close\nData: Cleanup\nExit", "State(s) in (\"\")"=w1014) -> ("States Out"=w1013:string)  [unwired: 1 in, 12 out]
      }
      frame "---------- Navigate ----------" {
      }
      frame "Navigate: Add" {
        n355 = Unbundle By Name(w1026) -> ("JKI SM"=w1021:refnum<class "JKI SM.lvclass">)
        n356 = call "Get All Case and Event Frames.vi"("error in (no error)"=w1020, "JKI SM in"=w1021) -> ("error out"=w1022:errorcluster, "Frame Names"=w1019:string[], "Frames[]"=w1023:refnum<vi>[])  [unwired: 1 in, 6 out]
        n357 = call "Search for Frame in Frames.vi"("Frame Name"=w1018, "Frame Names"=w1019) -> ("index of element"=w1025:i32)  [unwired: 9 in]
        n358 = Index Array(array=w1023, index=w1025) -> (element=w1024:refnum<vi>)
        n359 = in-place {
          in-place-border: w1024 -> [w1034]
          in-place-border: w1018 -> [w1029]
          n360 = in-place-cluster #1(w1026) -> ("NavHist"=w1032:refnum<vi>[], "NavIndex"=w1033:i32)  [unwired: 1 out]
          n361 = Increment(x=w1033) -> (x+1=w1031:i32)
          n362 = Reshape Array(w1032, w1031) -> (w1030:refnum<vi>[])
          n363 = Increment(x=w1033) -> (x+1=w1036:i32)
          n364 = Build Array (concatenate)(w1030, w1034) -> (w1035:refnum<vi>[])
          n365 = in-place-cluster #1("NavHist"=w1035, "NavIndex"=w1036, "tag"=w1029) -> (w1027:T13)
        }
      }
      frame "Navigation: Clear History" {
        n366 = Unbundle By Name(w1042) -> ("JKI SM"=w1040:refnum<class "JKI SM.lvclass">)
        n367 = call "Get All Case and Event Frames.vi"("error in (no error)"=w1038, "JKI SM in"=w1040) -> ("error out"=w1037:errorcluster, "Visible Frame"=w1039:refnum<vi>)  [unwired: 1 in, 7 out]
        n368 = Build Array(w1039) -> (w1043:refnum<vi>[])
        n369 = Bundle By Name(cluster=w1042, "NavHist"=w1043, "NavIndex"=0) -> (w1041:T13)
      }
      frame "---------- Scripting ----------" {
      }
      frame "Script: begin undo" {
        n370 = Unbundle By Name(w1057) -> ("CaseStrVI Ref"=w1050:refnum<vi>)
        n371 = property class="VI"(reference=w1050, error in=w1052) -> (reference out=w1049:refnum<vi>, error out=w1051:errorcluster, "Exec.State"=w1054:T16)
        n372 = case shown="\"Bad\", \"Idle\"" w1054 {
          tunnel: [w1060 w1065] -> w1058
          tunnel: w1056 -> [_ w1064]
          tunnel: w1051 -> [w1060 w1063]
          tunnel: w1049 -> [_ w1062]
          tunnel: [_ TRUE ("Undo Transaction")] -> w1053
          frame "Run top level", "Running" {
            # "Running, Don't allow undo"
          }
          frame "Bad", "Idle" {
            # "Not Running"
            n373 = invoke class="VI" method="Transaction.Begin Undo"(reference=w1062, error in=w1063, "Name"=w1064) -> (error out=w1065:errorcluster)  [unwired: 1 in, 3 out]
          }
        }
        n374 = Bundle By Name(cluster=w1057, "Undo Transaction"=w1053) -> (w1055:T13)
      }
      frame "Script: get CaseStruct ref" {
        w1068 = refnum<vi> refnum  # MultiFrameStructure
        # "I get the Active VI Ref from the RCF because I\nwant to implement Undo and I think I need that.\n\nGet the reference to the Case Structure here."
        n375 = Unbundle By Name(w1072) -> ("StructRef"=w1066:refnum<vi>)
        n376 = To More Specific Class(target class=w1068, reference=w1066, error in=w1070) -> (specific class reference=w1067:refnum<vi>, error out=w1069:errorcluster)
        n377 = Bundle By Name(cluster=w1072, "StructRef"=w1067) -> (w1071:T13)
      }
      frame "Script: get FrameNames" {
        w1086 = 1 items=["no exception", "cancel error on match", "set error on match"] ("[exception action] (none:0)")
        # "Why, oh why, did I put this here?\nI wish I commented it back then..."
        n378 = Unbundle By Name(w1091) -> ("JKI SM"=w1081:refnum<class "JKI SM.lvclass">, "Tree"=w1084:refnum<vi>)
        n379 = call "Get All Case and Event Frames.vi"("error in (no error)"=w1078, "JKI SM in"=w1081) -> ("error out"=w1077:errorcluster, "Frame Names"=w1080:string[], "Frames[]"=w1074:refnum<vi>[], "Visible Frame Index"=w1079:i32, "Num Event Frames"=w1076:i32)  [unwired: 1 in, 4 out]
        n380 = property class="Tree (strict)"(reference=w1084, error in=w1077) -> (error out=w1089:errorcluster, "DispItems"=w1083:string[], "TopLeft"=w1088:T11)  [unwired: 1 out]
        n381 = Unbundle By Name(w1088) -> ("Node"=w1075:string)
        n382 = call <vilib>:"General Error Handler.vi"("error in (no error)"=w1089, "[exception action] (none:0)"=w1086, "[exception code]"=1136) -> ("error out"=w1087:errorcluster)  [unwired: 2 in, 10 out]
        n383 = call "Search for Frame in Frames.vi"("Frame Name"=w1075, "Frame Names"=w1083) -> ("index of element"=w1082:i32)  [unwired: 9 in]
        n384 = Bundle By Name(cluster=w1091, "Num Event Frames"=w1076, "Frames[]"=w1074, "FrameNames"=w1080, "SelectedCase"=w1079, "Top Row Tag"=w1075, "Top Row Index"=w1082) -> (w1090:T13)
        n385 = call <vilib>:"Add State(s) to Queue__jki_lib_state_machine.vi"("State(s) in (\"\")"=w1093) -> ("States Out"=w1092:string)  [unwired: 2 in, 12 out]
      }
      frame "Script: check indent" {
        # "I only want to indent if the states\nin this Case Structure have section\nseparators (like the JKI SM).  Otherwise\nI'll put all items in the first col of the Tree."
        n386 = Unbundle By Name(w1102) -> ("FrameNames"=w1100:string[], "Core.Current VI Reference"=w1099:refnum<vi>)
        n387 = for {
          tunnel: w1100 -> [w1110] mode=indexing
          shift-right: [w1106] -> w1105
          shift-left: FALSE -> [w1107]
          n388 = Match Pattern(string=w1110, regular expression="-------") -> (offset past match=w1109:i32)  [unwired: 4 out]
          n389 = Greater Or Equal To 0?(x=w1109) -> (x >= 0?=w1108:bool)
          n390 = Or(x=w1108, y=w1107) -> (x .or. y?=w1106:bool)
        }
        n391 = property class="VI"(reference=w1099, error in=w1096) -> (error out=w1097:errorcluster, "Panel"=w1098:refnum<vi>)  [unwired: 1 out]
        n392 = property class="Pnl"(reference=w1098, error in=w1097, "DeferPanUpdts"=TRUE ("Defer Panel Updates")) -> (error out=w1095:errorcluster)  [unwired: 1 out]
        n393 = Bundle By Name(cluster=w1102, "Indent?"=w1105) -> (w1101:T13)
      }
      frame "Script: populate tree" {
        # "StructureTypes.ctlDO NOT CALL THIS FRAME DIRECTLY\nCALL \"Macro: update list\" instead, which will defer panel updates and other things"
        n394 = Unbundle By Name(w1116) -> ("Num Event Frames"=w1125:i32, "Indent?"=w1135:bool, "FrameNames"=w1120:string[], "TreeSectHdrs"=w1131:string, "Tree"=w1124:refnum<vi>)
        n395 = invoke class="Tree (strict)" method="Edit Tree Items.Delete"(reference=w1124, error in=w1134, "Delete Children"=TRUE ("Delete Children?")) -> (reference out=w1137:refnum<vi>, error out=w1127:errorcluster)  [unwired: 2 in, 3 out]
        n396 = Unbundle By Name(w1116) -> ("OpenCategoryFrames"=w1112:refnum<vi>[])
        n397 = call "JKI SM EDITOR - quick filter list.vi"("quick filter text"="Search", "Num Event Frames"=w1125, "States"=w1120, "error in"=w1127) -> ("States quick-filtered"=w1129:string[], "Indices quick-filtered"=w1118:i32[], "error out"=w1126:errorcluster)  [unwired: 8 in, 1 out]
        n398 = Unbundle By Name(w1116) -> ("Frames[]"=w1113:refnum<vi>[], "FrameNames"=w1114:string[])
        n399 = call "Search for Frame in Frames.vi"("Frame Name"="\"\"", "Frame Names"=w1120) -> ("index of element"=w1119:i32)  [unwired: 9 in]
        n400 = for {
          tunnel: w1131 -> [w1165]
          tunnel: w1135 -> [w1164]
          tunnel: w1129 -> [w1150] mode=indexing
          shift-right: [w1157] -> w1123
          shift-left: w1137 -> [w1171]
          shift-right: [w1166] -> w1122
          shift-left: w1126 -> [w1163]
          tunnel: w1125 -> [w1161]
          tunnel: w1118 -> [w1158] mode=indexing
          tunnel: w1119 -> [w1156]
          shift-right: [w1153] -> _
          shift-left: FALSE -> [w1154]
          tunnel: [w1150] -> w1115 mode=indexing if=w1149
          i -> [w1159]
          # "Don't indent the first case."
          # "Fill the Tree"
          n401 = Match Pattern(string=w1150, regular expression=w1165) -> (offset past match=w1170:i32)  [unwired: 4 out]
          n402 = Less Than 0?(x=w1170) -> (x < 0?=w1152:bool)
          n403 = Not Equal To 0?(x=w1159) -> (x != 0?=w1155:bool)
          n404 = Or(x=w1154, y=w1152) -> (x .or. y?=w1153:bool)
          n405 = Compound Arithmetic op=AND(w1164, w1152, w1155) -> (w1151:bool)
          n406 = call "Is An Event Frame.vi"("Event Structure index"=w1156, "index of element"=w1158, "Num Event Frames"=w1161) -> ("Structure Type"=w1160:T17)  [unwired: 7 in, 1 out]
          n407 = call "Treat Frame Name for Dialog.vi"("Selected Structure"=w1160, "index of element"=w1158, "Frame Name (tag)"=w1150) -> ("Frame Name for Dialog"=w1162:string)  [unwired: 8 in]
          n408 = Select(t=1 ("New Item Indentation"), s=w1151, f=0 ("New Item Indentation")) -> (s? t:f=w1167:i32)
          n409 = invoke class="Tree (strict)" method="Edit Tree Items.Add Item to End"(reference=w1171, error in=w1163, "Left Cell"=w1162, "Child Tag"=w1150, "Item Indent"=w1167) -> (reference out=w1157:refnum<vi>, error out=w1166:errorcluster)  [unwired: 3 in, 6 out]
          n410 = Not(x=w1151) -> (.not. x?=w1149:bool)
        }
        n411 = for {
          tunnel: w1115 -> [w1140] mode=indexing
          tunnel: w1114 -> [w1148]
          tunnel: w1113 -> [w1146]
          tunnel: w1112 -> [w1145]
          tunnel: w1123 -> [w1142]
          n412 = Search 1D Array(1D array=w1148, element=w1140) -> (index of element=w1147:i32)  [unwired: 1 in]
          n413 = Index Array(array=w1146, index=w1147) -> (element=w1144:refnum<vi>)
          n414 = Search 1D Array(1D array=w1145, element=w1144) -> (index of element=w1143:i32)  [unwired: 1 in]
          n415 = Greater Or Equal To 0?(x=w1143) -> (x >= 0?=w1141:bool)
          n416 = invoke class="Tree (strict)" method="Open/Close.Item"(reference=w1142, "tag"=w1140, "Open"=w1141) -> ()  [unwired: 2 in, 5 out]
        }
        n417 = property class="Tree (strict)"(reference=w1123, error in=w1122) -> (error out=w1128:errorcluster, "DispItems"=w1138:string[])  [unwired: 1 out]
        n418 = Array Size(array=w1138) -> (size(s)=w1139:i32)
        n419 = Bundle By Name(cluster=w1116, "DisplayedItems"=w1139) -> (w1132:T13)
      }
      frame "Script: select case" {
        n420 = Unbundle By Name(w1187) -> ("JKI SM"=w1179:refnum<class "JKI SM.lvclass">, "tag"=w1178:string)
        n421 = call "Get All Case and Event Frames.vi"("error in (no error)"=w1177, "JKI SM in"=w1179) -> ("error out"=w1176:errorcluster, "Frame Names"=w1181:string[], "Visible Frame Name"=w1180:string, "Num Event Frames"=w1175:i32, "Event Frame Index"=w1172:i32)  [unwired: 1 in, 4 out]
        n422 = Not Equal?(x=w1178, y=w1180) -> (x != y?=w1182:bool)
        n423 = call "Search for Frame in Frames.vi"("Frame Name"=w1178, "Frame Names"=w1181) -> ("index of element"=w1174:i32)  [unwired: 9 in]
        n424 = call "Is An Event Frame.vi"("Event Structure index"=w1172, "index of element"=w1174, "Num Event Frames"=w1175) -> ("Event Frame?"=w1173:bool)  [unwired: 7 in, 1 out]
        n425 = case shown="True" w1182 {
          tunnel: [w1189 w1192] -> w1185
          tunnel: w1176 -> [w1189 w1193]
          tunnel: w1174 -> [_ w1191]
          tunnel: w1173 -> [_ w1196]
          tunnel: w1179 -> [_ w1195]
          tunnel: w1178 -> [_ w1194]
          frame False {
          }
          frame True {
            n426 = Decrement(x=w1191) -> (x-1=w1190:i32)
            n427 = call "Set Visible State.vi"("Event Structure Frame (-1: Use State Name)"=w1190, "Event Structure (F: Case Structure)"=w1196, "error in (no error)"=w1193, "State Name"=w1194, "JKI SM in"=w1195) -> ("error out"=w1192:errorcluster)  [unwired: 5 in, 1 out]
          }
        }
        n428 = Bundle By Name(cluster=w1187, "SelectedCase"=w1174) -> (w1183:T13)
        n429 = Unbundle By Name(w1185) -> ("code"=w1184:i32)
        n430 = case shown="1" w1184 {
          tunnel: [w1197 w1199 w1200] -> w1186
          tunnel: w1185 -> [w1197 w1198 w1200]
          frame 0, Default {
          }
          frame 1 {
            # "Ignore error after drag/copy operation."
            n431 = call <vilib>:"Clear Errors.vi"("error in (no error)"=w1198) -> ("error out"=w1199:errorcluster)  [unwired: 1 in, 5 out]
          }
          frame 1055 {
            # "Invalid reference"
          }
        }
      }
      frame "Script: sort list" {
        n432 = Unbundle By Name(w1208) -> ("StructRef"=w1201:refnum<vi>, "FrameNames"=w1203:string[], "TreeSectHdrs"=w1202:string)
        n433 = call "SortAlphabetically.vi"("error in"=w1206, "TreeSectHdrs"=w1202, "FrameNames"=w1203) -> ("error out"=w1205:errorcluster, "Sorted"=w1204:i32[])  [unwired: 7 out]
        n434 = invoke class="MFStruct" method="RearrangeFramesByIdx"(reference=w1201, error in=w1205, "Index Array"=w1204) -> (error out=w1207:errorcluster)  [unwired: 1 in, 3 out]
      }
      frame "Script: Add Dynamic Events" {
        n435 = Unbundle By Name(w1213) -> ("JKI SM"=w1210:refnum<class "JKI SM.lvclass">)
        n436 = call-dynamic "Add Event Registration Category.vi"("error in (no error)"=w1212, "JKI SM in"=w1210) -> ("error out"=w1211:errorcluster)  [unwired: 8 in, 1 out]
      }
      frame "Script: delete frame" {
        # "commented this out"
        # "Don't need to do full tree refresh if we delete single item in tree here."
        n437 = Unbundle By Name(w1225) -> ("FrameNames"=w1220:string[], "JKI SM"=w1224:refnum<class "JKI SM.lvclass">, "Tree"=w1216:refnum<vi>, "Num Event Frames"=w1215:i32)
        n438 = Empty String/Path?(string/path=w1217) -> (empty?=w1218:bool)
        n439 = case shown="False" w1218 {
          tunnel: w1226 -> [w1252 w1286]
          tunnel: w1224 -> [w1250 _]
          tunnel: w1220 -> [w1229 _]
          tunnel: [w1244 w1286] -> w1219
          tunnel: w1217 -> [w1235 _]
          tunnel: w1216 -> [w1236 _]
          tunnel: w1215 -> [w1232 _]
          frame False {
            # "Find 1st case\nw/o a name"
            n440 = call "Parse State from Frame Name.vi"("Frame or State Name"=w1235) -> ("is a Category Frame?"=w1237:bool, "Category Name"=w1238:string)  [unwired: 5 in, 4 out]
            n441 = Select(t=w1238, s=w1237, f=w1235) -> (s? t:f=w1234:string)
            n442 = call "Search for Frame in Frames.vi"("Frame Name"="", "Frame Names"=w1229) -> ("index of element"=w1246:i32)  [unwired: 9 in]
            n443 = call "Search for Frame in Frames.vi"("Frame Name"=w1235, "Frame Names"=w1229) -> ("index of element"=w1231:i32)  [unwired: 9 in]
            n444 = call "Search for Frame in Frames.vi"("Frame Name"="\"\"", "Frame Names"=w1229) -> ("index of element"=w1227:i32)  [unwired: 9 in]
            n445 = Less Than 0?(x=w1231) -> (x < 0?=w1247:bool)
            n446 = call "Is An Event Frame.vi"("Event Structure index"=w1227, "index of element"=w1231, "Num Event Frames"=w1232) -> ("Structure Type"=w1230:T17)  [unwired: 7 in, 1 out]
            n447 = case shown="\"EventStructure\"" w1230 {
              tunnel: ["Delete %s state frame and all callers?\n(use Find Callers if unsure)" ("format string") "Delete \"%s\" event frame?" ("format string")] -> w1240
              frame "CaseStructure" {
              }
              frame "EventStructure" {
              }
            }
            n448 = call "Treat Frame Name for Dialog.vi"("Selected Structure"=w1230, "index of element"=w1231, "Frame Name (tag)"=w1234) -> ("Frame Name for Dialog"=w1233:string)  [unwired: 8 in]
            n449 = Select(t="", s=w1247, f=w1233) -> (s? t:f=w1242:string)
            n450 = Select(t=w1246, s=w1247, f=w1231) -> (s? t:f=w1245:i32)
            n451 = Select(t="Delete \"%s\" category?" ("format string"), s=w1237, f=w1240) -> (s? t:f=w1239:string)
            n452 = Format Into String(format string=w1239, w1242) -> (resulting string=w1251:string)  [unwired: 2 in, 1 out]
            n453 = Two Button Dialog(message=w1251) -> (T button?=w1243:bool)  [unwired: 2 out]
            n454 = case shown="True" w1243 {
              tunnel: w1252 -> [w1255 w1267]
              tunnel: [w1255 w1256] -> w1244
              tunnel: w1250 -> [_ w1266]
              tunnel: w1245 -> [_ w1265]
              tunnel: w1230 -> [_ w1263]
              tunnel: w1242 -> [_ w1262]
              tunnel: w1237 -> [_ w1261]
              tunnel: w1236 -> [_ w1258]
              tunnel: w1235 -> [_ w1259]
              frame False {
              }
              frame True {
                w1260 = FALSE  # Delete Children?
                # "Delete Item"
                n455 = To Unsigned Long Integer(number=w1265) -> (unsigned 32bit integer=w1264:u32)
                n456 = case shown="\"EventStructure\"" w1263 {
                  tunnel: w1267 -> [w1270 w1279]
                  tunnel: [w1268 w1284] -> w1257
                  tunnel: w1266 -> [w1269 w1281]
                  tunnel: w1264 -> [_ w1283]
                  tunnel: w1263 -> [_ w1282]
                  tunnel: w1262 -> [w1274 _]
                  tunnel: w1261 -> [w1275 _]
                  tunnel: w1259 -> [_ _]
                  frame "CaseStructure" {
                    n457 = Swap Values(12:"", 13:w1275, 14:w1274) -> (1:w1271:string, 3:w1273:string)
                    n458 = call "Delete State.vi"("Delete Callers? (F: Only Delete Case Structure Frame)"=TRUE, "error in (no error)"=w1270, "State Name"=w1273, "Category (Optional)"=w1271, "JKI SM in"=w1269) -> ("error out"=w1268:errorcluster)  [unwired: 5 in, 1 out]
                  }
                  frame "EventStructure" {
                    n459 = Decrement(x=w1283) -> (x-1=w1277:u32)
                    n460 = call "Get VI Event Structure Reference.vi"("error in (no error)"=w1279, "JKI SM in"=w1281) -> ("error out"=w1278:errorcluster, "Event Structure ref"=w1280:refnum<vi>)  [unwired: 7 in, 1 out]
                    n461 = call "Script - delete frame.vi"("errorin"=w1278, "Structure Type"=w1282, "Frame Index"=w1277, "StructRef"=w1280) -> ("error out"=w1284:errorcluster)  [unwired: 7 in]
                  }
                }
                n462 = invoke on="Tree: Delete Item" class="Tree (strict)" method="Edit Tree Items.Delete"(reference=w1258, error in=w1257, "tag"=w1259, "Delete Children"=w1260) -> (error out=w1256:errorcluster)  [unwired: 1 in, 4 out]
              }
            }
          }
          frame True {
            n463 = One Button Dialog(message="You need to select a case first.") -> ()  [unwired: 2 out]
          }
        }
        n464 = call <vilib>:"Add State(s) to Queue__jki_lib_state_machine.vi"("State(s) in Front (\"\")"="// Macro: update list" ("State(s) in Front (\"\")"), "State(s) in (\"\")"=w1223) -> ("States Out"=w1222:string)  [unwired: 1 in, 12 out]
      }
      frame "Script: insert frame" {
        n465 = Unbundle By Name(w1308) -> ("FrameNames"=w1302:string[], "JKI SM"=w1298:refnum<class "JKI SM.lvclass">)
        n466 = call "Parse State from Frame Name.vi"("Frame or State Name"=w1299) -> ("Category Name"=w1300:string)  [unwired: 5 in, 5 out]
        n467 = call "Search for Frame in Frames.vi"("Frame Name"=w1299, "Frame Names"=w1302) -> ("index of element"=w1306:i32)  [unwired: 9 in]
        n468 = Array Size(array=w1302) -> (size(s)=w1294:i32)
        n469 = Less Than 0?(x=w1306) -> (x < 0?=w1295:bool)
        n470 = call "Get All Case and Event Frames.vi"("error in (no error)"=w1297, "JKI SM in"=w1298) -> ("error out"=w1293:errorcluster, "Num Event Frames"=w1291:i32, "Event Frame Index"=w1287:i32)  [unwired: 1 in, 6 out]
        n471 = Select(t=w1294, s=w1295, f=w1306) -> (s? t:f=w1290:i32)
        n472 = call "Is An Event Frame.vi"("Event Structure index"=w1287, "index of element"=w1290, "Num Event Frames"=w1291) -> ("Structure Type"=w1288:T17, "Event Frame?"=w1289:bool)  [unwired: 7 in]
        n473 = call "PromptUserWithDefault.vi"("Structure Type"=w1288, "Section"=w1300) -> ("OK"=w1292:bool, "NewTag 2"=w1301:string)  [unwired: 2 in, 6 out]
        n474 = Insert Into Array(array=w1302, index=w1290, new element=w1301) -> (w1296:string[])
        n475 = case shown="True" w1292 {
          tunnel: [w1309 w1318] -> w1307
          tunnel: w1306 -> [_ w1317]
          tunnel: w1301 -> [_ w1316]
          tunnel: w1299 -> [_ w1315]
          tunnel: w1298 -> [_ w1314]
          tunnel: w1296 -> [_ w1313]
          tunnel: w1290 -> [_ w1312]
          tunnel: w1293 -> [w1309 w1311]
          tunnel: w1289 -> [_ w1310]
          frame False {
            # "User cancelled the operation."
          }
          frame True {
            n476 = case shown="True" w1310 {
              tunnel: w1311 -> [w1325 w1328]
              tunnel: w1314 -> [w1319 w1331]
              tunnel: [w1324 w1329] -> w1318
              tunnel: w1313 -> [_ _]
              tunnel: w1317 -> [_ w1332]
              tunnel: w1316 -> [w1320 _]
              tunnel: w1312 -> [_ _]
              tunnel: w1315 -> [w1323 _]
              frame False {
                # "Case Structure"
                n477 = call "Add New State.vi"("After State (Optional)"=w1323, "error in (no error)"=w1325, "State Name"=w1320, "JKI SM in"=w1319) -> ("error out"=w1321:errorcluster, "JKI SM out"=w1322:refnum<class "JKI SM.lvclass">)  [unwired: 5 in, 1 out]
                n478 = call "Set Visible State.vi"("error in (no error)"=w1321, "State Name"=w1320, "JKI SM in"=w1322) -> ("error out"=w1324:errorcluster)  [unwired: 7 in, 1 out]
              }
              frame True {
                # "Event Structure frames are offset by 1 (under \"Idle\")"
                # "Event Structure"
                n479 = call "Get VI Event Structure Reference.vi"("error in (no error)"=w1328, "JKI SM in"=w1331) -> ("error out"=w1327:errorcluster, "Event Structure ref"=w1330:refnum<vi>)  [unwired: 7 in, 1 out]
                n480 = Increment(x=w1332) -> (x+1=w1326:i32)
                n481 = To Unsigned Long Integer(number=w1326) -> (unsigned 32bit integer=w1334:u32)
                n482 = invoke class="EvntStruct" method="Add Frame"(reference=w1330, error in=w1327, "Reference Frame Index"=w1334, "After? (T)"=FALSE) -> (error out=w1329:errorcluster)  [unwired: 1 in, 4 out]
              }
            }
          }
        }
        n483 = call <vilib>:"Add State(s) to Queue__jki_lib_state_machine.vi"("State(s) in Front (\"\")"="Macro: update list" ("State(s) in Front (\"\")"), "State(s) in (\"\")"=w1305) -> ("States Out"=w1304:string)  [unwired: 1 in, 12 out]
      }
      frame "Script: rename case" {
        n484 = Unbundle By Name(w1344) -> ("Tree"=w1342:refnum<vi>, "JKI SM"=w1350:refnum<class "JKI SM.lvclass">, "Num Event Frames"=w1341:i32, "FrameNames"=w1336:string[])
        n485 = call "Search for Frame in Frames.vi"("Frame Name"=w1340, "Frame Names"=w1336) -> ("index of element"=w1339:i32)  [unwired: 9 in]
        n486 = call "Parse State from Frame Name.vi"("Frame or State Name"=w1340) -> ("is a Category Frame?"=w1348:bool, "State Name"=w1346:string, "Category Name"=w1347:string, "\"Category: State\" String"=w1345:string)  [unwired: 5 in, 2 out]
        n487 = call "Search for Frame in Frames.vi"("Frame Name"="\"\"", "Frame Names"=w1336) -> ("index of element"=w1335:i32)  [unwired: 9 in]
        n488 = call "Is An Event Frame.vi"("Event Structure index"=w1335, "index of element"=w1339, "Num Event Frames"=w1341) -> ("Structure Type"=w1338:T17)  [unwired: 7 in, 1 out]
        n489 = case shown="\"CaseStructure\", Default" w1338 {
          tunnel: [w1366 w1383] -> w1352
          tunnel: w1347 -> [w1365 _]
          tunnel: w1340 -> [w1364 _]
          tunnel: w1350 -> [w1363 _]
          tunnel: w1349 -> [w1362 w1383]
          tunnel: w1346 -> [w1361 _]
          tunnel: w1348 -> [w1360 _]
          tunnel: w1347 -> [w1358 _]
          tunnel: w1346 -> [w1357 _]
          tunnel: w1345 -> [w1356 _]
          tunnel: w1344 -> [w1355 w1382]
          tunnel: [w1354 w1382] -> w1343
          tunnel: w1340 -> [w1353 _]
          tunnel: w1342 -> [_ _]
          frame "CaseStructure", Default {
            n490 = call "PromptUserWithDefault.vi"("is Category?"=w1360, "Recommended Name (\"\": None)"=w1361, "Section"=w1365) -> ("OK"=w1359:bool, "NewTag 2"=w1367:string)  [unwired: 1 in, 6 out]
            n491 = case shown="True" w1359 {
              tunnel: w1367 -> [_ w1373]
              tunnel: [w1369 w1370] -> w1366
              tunnel: w1364 -> [_ _]
              tunnel: w1363 -> [_ w1371]
              tunnel: w1362 -> [w1369 w1381]
              tunnel: w1358 -> [_ w1380]
              tunnel: w1357 -> [_ w1379]
              tunnel: w1356 -> [_ _]
              tunnel: w1355 -> [w1368 w1374]
              tunnel: [w1368 w1374] -> w1354
              tunnel: w1353 -> [_ _]
              frame False {
              }
              frame True {
                n492 = call "Parse State from Frame Name.vi"("Wrap in Quotes? (FALSE)"=TRUE, "Frame or State Name"=w1373) -> ("State Name"=w1377:string, "Category Name"=w1378:string)  [unwired: 4 in, 4 out]
                n493 = call "Get VI Reference.vi"("error in (no error)"=w1381, "JKI SM in"=w1371) -> ("error out"=w1375:errorcluster, "JKI SM out"=w1376:refnum<class "JKI SM.lvclass">)  [unwired: 7 in, 1 out]
                n494 = call-dynamic "Rename State.vi"("Category"=w1380, "State"=w1379, "error in (no error)"=w1375, "New State"=w1377, "New Category (\"\": Use Existing)"=w1378, "JKI SM in"=w1376) -> ("error out"=w1370:errorcluster)  [unwired: 2 in, 3 out]
              }
            }
          }
          frame "EventStructure" {
            # "renaming cases doesn't apply to Event Structures"
          }
        }
      }
      frame "Script: duplicate case" {
        n495 = Unbundle By Name(w1400) -> ("Num Event Frames"=w1388:i32, "FrameNames"=w1385:string[], "JKI SM"=w1395:refnum<class "JKI SM.lvclass">)
        n496 = call "Search for Frame in Frames.vi"("Frame Name"=w1390, "Frame Names"=w1385) -> ("index of element"=w1389:i32)  [unwired: 9 in]
        n497 = call "Search for Frame in Frames.vi"("Frame Name"="\"\"", "Frame Names"=w1385) -> ("index of element"=w1384:i32)  [unwired: 9 in]
        n498 = call "Is An Event Frame.vi"("Event Structure index"=w1384, "index of element"=w1389, "Num Event Frames"=w1388) -> ("Structure Type"=w1387:T17)  [unwired: 7 in, 1 out]
        n499 = call "Parse State from Frame Name.vi"("Frame or State Name"=w1390) -> ("is a Category Frame?"=w1391:bool, "State Name"=w1392:string, "Category Name"=w1393:string)  [unwired: 5 in, 3 out]
        n500 = case shown="\"CaseStructure\", Default" w1387 {
          tunnel: w1385 -> [w1418 w1440]
          tunnel: [w1414 w1433] -> w1399
          tunnel: w1393 -> [w1407 _]
          tunnel: [w1413 ""] -> w1396
          tunnel: w1390 -> [w1412 w1438]
          tunnel: w1395 -> [w1401 w1430]
          tunnel: w1394 -> [w1411 w1432]
          tunnel: w1392 -> [w1410 _]
          tunnel: w1391 -> [w1402 _]
          frame "CaseStructure", Default {
            n501 = Swap Values(12:"", 13:w1402, 14:" (copy)" ("string")) -> (1:w1403:string, 3:w1404:string)
            n502 = Concatenate Strings(w1410, w1404) -> (w1409:string)
            n503 = Concatenate Strings(w1407, w1403) -> (w1408:string)
            n504 = call "Search for Frame in Frames.vi"("Frame Name"=w1412, "Frame Names"=w1418) -> ("index of element"=w1417:i32)  [unwired: 9 in]
            n505 = call "PromptUserWithDefault.vi"("is Category?"=w1402, "Recommended Name (\"\": None)"=w1409, "Section"=w1408) -> ("OK"=w1415:bool, "NewTag 2"=w1416:string)  [unwired: 1 in, 6 out]
            n506 = case shown="True" w1415 {
              tunnel: w1418 -> [_ _]
              tunnel: w1417 -> [_ _]
              tunnel: w1416 -> [_ w1424]
              tunnel: w1411 -> [w1419 w1427]
              tunnel: [w1419 w1423] -> w1414
              tunnel: w1401 -> [_ w1426]
              tunnel: [_ ""] -> w1413
              tunnel: w1412 -> [_ w1422]
              frame False {
              }
              frame True {
                n507 = call-dynamic "Duplicate State.vi"("State to Duplicate"=w1422, "error in (no error)"=w1427, "New State"=w1424, "JKI SM in"=w1426) -> ("error out"=w1421:errorcluster, "JKI SM out"=w1420:refnum<class "JKI SM.lvclass">)  [unwired: 6 in]
                n508 = call "Set Visible State.vi"("error in (no error)"=w1421, "State Name"=w1424, "JKI SM in"=w1420) -> ("error out"=w1423:errorcluster)  [unwired: 7 in, 1 out]
              }
            }
          }
          frame "EventStructure" {
            # "Event Structure Frames are offset by 1 (underneath \"Idle\")"
            n509 = call "Search for Frame in Frames.vi"("Frame Name"=w1438, "Frame Names"=w1440) -> ("index of element"=w1436:i32)  [unwired: 9 in]
            n510 = call "Get VI Event Structure Reference.vi"("error in (no error)"=w1432, "JKI SM in"=w1430) -> ("error out"=w1429:errorcluster, "Event Structure ref"=w1431:refnum<vi>)  [unwired: 7 in, 1 out]
            n511 = Decrement(x=w1436) -> (x-1=w1428:i32)
            n512 = invoke class="EvntStruct" method="Duplicate Frame"(reference=w1431, error in=w1429, "Frame Index"=w1428) -> (reference out=w1437:refnum<vi>, error out=w1434:errorcluster)  [unwired: 1 in, 2 out]
            n513 = Increment(x=w1428) -> (x+1=w1435:i32)
            n514 = property class="EvntStruct"(reference=w1437, error in=w1434, "VisFrame"=w1435) -> (error out=w1433:errorcluster)  [unwired: 1 out]
          }
        }
        n515 = call <vilib>:"Add State(s) to Queue__jki_lib_state_machine.vi"("State(s) in Front (\"\")"=w1396, "State(s) in (\"\")"=w1398) -> ("States Out"=w1397:string)  [unwired: 13 in]
      }
      frame "Script: Find Callers" {
        n516 = Unbundle By Name(w1458) -> ("Num Event Frames"=w1447:i32, "FrameNames"=w1443:string[], "JKI SM"=w1453:refnum<class "JKI SM.lvclass">)
        n517 = call "Parse State from Frame Name.vi"("Frame or State Name"=w1445) -> ("is a Category Frame?"=w1449:bool, "State Name"=w1450:string, "Category Name"=w1451:string)  [unwired: 5 in, 3 out]
        n518 = call "Search for Frame in Frames.vi"("Frame Name"=w1445, "Frame Names"=w1443) -> ("index of element"=w1446:i32)  [unwired: 9 in]
        n519 = call "Search for Frame in Frames.vi"("Frame Name"="\"\"", "Frame Names"=w1443) -> ("index of element"=w1442:i32)  [unwired: 9 in]
        n520 = call "Is An Event Frame.vi"("Event Structure index"=w1442, "index of element"=w1446, "Num Event Frames"=w1447) -> ("Structure Type"=w1448:T17)  [unwired: 7 in, 1 out]
        n521 = case shown="\"CaseStructure\", Default" w1448 {
          tunnel: w1443 -> [_ _]
          tunnel: [w1464 w1468] -> w1457
          tunnel: w1451 -> [_ _]
          tunnel: [_ ""] -> w1454
          tunnel: w1445 -> [w1463 _]
          tunnel: w1453 -> [w1461 _]
          tunnel: w1452 -> [w1467 w1468]
          tunnel: w1450 -> [_ _]
          tunnel: w1449 -> [_ _]
          tunnel: w1441 -> [w1460 _]
          frame "CaseStructure", Default {
            n522 = call "Find All Callers of State.vi"("error in (no error)"=w1467, "State Name"=w1463, "JKI SM in"=w1461) -> ("error out"=w1465:errorcluster, "Callers"=w1466:T18)  [unwired: 6 in, 1 out]
            n523 = call "Get VI Case Structure Reference.vi"("JKI SM in"=w1461) -> ("Case Structure ref"=w1462:refnum<vi>)  [unwired: 8 in, 2 out]
            n524 = call "Get Calling VI Details.vi"("User VI Ref"=w1460, "Affected Items"=w1462) -> ("Calling VI Details"=w1459:T5)  [unwired: 9 in]
            n525 = call "Open Search Results Dialog.vi"("error in (no error)"=w1465, "Callers"=w1466, "State"=w1463, "Calling VI Details"=w1459) -> ("error out"=w1464:errorcluster)  [unwired: 7 in]
          }
          frame "EventStructure" {
          }
        }
        n526 = call <vilib>:"Add State(s) to Queue__jki_lib_state_machine.vi"("State(s) in Front (\"\")"=w1454, "State(s) in (\"\")"=w1456) -> ("States Out"=w1455:string)  [unwired: 13 in]
      }
      frame "Script: rename strings in VI" {
        # "Replace all calls to the old state name with the new one."
        n527 = Unbundle By Name(w1486) -> ("CaseStrVI Ref"=w1481:refnum<vi>)
        n528 = Match Pattern(string=w1478, regular expression=",") -> (before substring=w1472:string, after substring=w1474:string)  [unwired: 1 in, 2 out]
        n529 = Search and Replace String(replace all?=TRUE ("replace all? (F)"), input string=w1472, search string="\"") -> (result string=w1471:string)  [unwired: 5 in, 3 out]
        n530 = call <vilib>:"TRef Traverse for References.vi"("Traverse Target"=TRef_TravTarget."BD", "error in (no error)"=w1476, "Class Name"="StringConstant", "VI Refnum"=w1481) -> ("error out"=w1479:errorcluster, "References"=w1480:refnum<vi>[])  [unwired: 1 in, 5 out]
        n531 = for {
          tunnel: w1480 -> [w1506] mode=indexing
          tunnel: w1479 -> [w1503]
          tunnel: w1471 -> [w1489]
          tunnel: w1474 -> [w1488]
          tunnel: [w1491] -> w1475
          w1504 = refnum<vi> refnum  # StringConstant
          n532 = To More Specific Class(target class=w1504, reference=w1506, error in=w1503) -> (specific class reference=w1505:refnum<vi>, error out=w1502:errorcluster)
          n533 = property class="StrCnst"(reference=w1505, error in=w1502) -> (reference out=w1495:refnum<vi>, error out=w1498:errorcluster, "Value"=w1501:variant)
          n534 = Variant To Data(error in=w1498, type="", Variant=w1501) -> (data=w1490:string, error out=w1499:errorcluster)
          n535 = Search and Replace String(replace all?=TRUE ("replace all? (F)"), input string=w1490, search string=w1489, replace string=w1488, error in=w1499) -> (result string=w1487:string, error out=w1496:errorcluster)  [unwired: 3 in, 2 out]
          n536 = To Variant(anything=w1487) -> (Variant=w1494:variant)
          n537 = property class="StrCnst"(reference=w1495, error in=w1496, "Value"=w1494) -> (reference out=w1492:refnum<vi>, error out=w1493:errorcluster)
          n538 = Close Reference(reference=w1492, error in (no error)=w1493) -> (error out=w1491:errorcluster)
        }
        n539 = call <vilib>:"Add State(s) to Queue__jki_lib_state_machine.vi"("State(s) in (\"\")"=w1485) -> ("States Out"=w1484:string)  [unwired: 14 in]
      }
      frame "Script: process drag-copy" {
        # "New frame index >>"
        # "Index of original frame"
        # "Find case name"
        n540 = Unbundle By Name(w1521) -> ("FrameNames"=w1517:string[], "Tree"=w1520:refnum<vi>)
        n541 = property class="Tree (strict)"(reference=w1520, error in=w1519) -> (error out=w1515:errorcluster, "All Tags"=w1508:string[])  [unwired: 1 out]
        n542 = for {
          tunnel: w1508 -> [w1527] mode=indexing
          tunnel: w1517 -> [w1528]
          shift-right: [w1522] -> w1512
          shift-left: 0 -> [w1524]
          i -> [w1523]
          # "Find new case"
          n543 = call "Search for Frame in Frames.vi"("Frame Name"=w1527, "Frame Names"=w1528) -> ("index of element"=w1526:i32)  [unwired: 9 in]
          n544 = Greater Than 0?(x=w1526) -> (x > 0?=w1525:bool)
          n545 = Select(t=w1524, s=w1525, f=w1523) -> (s? t:f=w1522:i32)
        }
        n546 = Bundle By Name(cluster=w1521, "FrameNames"=w1508) -> (w1509:T13)
        n547 = Index Array(array=w1508, index=w1512) -> (element=w1516:string)
        n548 = call "Search for Frame in Frames.vi"("Frame Name"=w1516, "Frame Names"=w1517) -> ("index of element"=w1513:i32)  [unwired: 9 in]
        n549 = Format Into String(format string="Macro: copy frame >> %d,%d", w1513, w1512) -> (resulting string=w1507:string)  [unwired: 2 in, 1 out]
        n550 = call <vilib>:"Add State(s) to Queue__jki_lib_state_machine.vi"("State(s) in Front (\"\")"=w1507, "State(s) in (\"\")"=w1511) -> ("States Out"=w1510:string)  [unwired: 1 in, 12 out]
      }
      frame "Script: copy frame" {
        n551 = Unbundle By Name(w1551) -> ("Num Event Frames"=w1533:i32, "SectHdr"=w1542:string, "FrameNames"=w1530:string[], "StructRef"=w1550:refnum<vi>)
        n552 = call "Search for Frame in Frames.vi"("Frame Name"=w1535, "Frame Names"=w1530) -> ("index of element"=w1534:i32)  [unwired: 9 in]
        n553 = call "Search for Frame in Frames.vi"("Frame Name"="\"\"", "Frame Names"=w1530) -> ("index of element"=w1529:i32)  [unwired: 9 in]
        n554 = call "Is An Event Frame.vi"("Event Structure index"=w1529, "index of element"=w1534, "Num Event Frames"=w1533) -> ("Structure Type"=w1532:T17)  [unwired: 7 in, 1 out]
        n555 = Scan From String(format string="%d,%d", input string=w1535) -> (output 1=w1547:i32, output 2=w1548:i32)  [unwired: 2 in, 5 out]
        n556 = call "PromptUserWithDefault.vi"("Structure Type"=w1532, "Section"=w1542) -> ("OK"=w1543:bool, "NewTag 2"=w1539:string)  [unwired: 2 in, 6 out]
        n557 = Format Into String(format string="\"%s\"", w1539) -> (resulting string=w1538:string)  [unwired: 2 in, 1 out]
        n558 = case shown="True" w1543 {
          tunnel: w1550 -> [_ w1566]
          tunnel: w1548 -> [_ w1555]
          tunnel: w1547 -> [_ w1565]
          tunnel: w1536 -> [w1552 w1564]
          tunnel: w1530 -> [_ w1557]
          tunnel: w1539 -> [_ w1556]
          tunnel: [w1552 w1558] -> w1537
          tunnel: w1532 -> [_ w1553]
          frame False {
            # "User cancelled the operation."
          }
          frame True {
            n559 = for {
              tunnel: [w1567] -> w1559 mode=indexing
              tunnel: w1557 -> [_] mode=indexing
              i -> [w1567]
            }
            n560 = Increment(x=w1565) -> (x+1=w1562:i32)
            n561 = Delete From Array(array=w1559, index=w1562) -> (deleted portion=w1561:i32, array with subset deleted=w1563:i32[])  [unwired: 1 in]
            n562 = Insert Into Array(array=w1563, index=w1555, new element=w1561) -> (w1560:i32[])
            n563 = Replace Array Subset(array=w1557, new element=w1556, index=w1555) -> (w1554:string[])
            n564 = call "Script - copy frame.vi"("FrameNames"=w1554, "Array"=w1560, "error in"=w1564, "Structure Type"=w1553, "Numeric"=w1565, "StructRef"=w1566) -> ("error out"=w1558:errorcluster)  [unwired: 5 in]
          }
        }
        n565 = Bundle By Name(cluster=w1551, "tag"=w1538) -> (w1541:T13)
        n566 = call <vilib>:"Add State(s) to Queue__jki_lib_state_machine.vi"("State(s) in Front (\"\")"="Macro: update list\nMacro: update list" ("State(s) in Front (\"\")"), "State(s) in (\"\")"=w1546) -> ("States Out"=w1545:string)  [unwired: 1 in, 12 out]
      }
      frame "Script: drop state name" {
      }
      frame "Script: end undo" {
        n567 = Unbundle By Name(w1577) -> ("Undo Transaction"=w1571:bool, "CaseStrVI Ref"=w1575:refnum<vi>)
        n568 = case shown="True" w1571 {
          tunnel: w1576 -> [w1579 w1582]
          tunnel: w1575 -> [_ w1581]
          tunnel: [w1579 w1580] -> w1574
          frame False {
          }
          frame True {
            n569 = invoke class="VI" method="Transaction.End Undo"(reference=w1581, error in=w1582) -> (error out=w1583:errorcluster)  [unwired: 1 in, 2 out]
            n570 = call <vilib>:"Clear Errors.vi"("error in (no error)"=w1583) -> ("error out"=w1580:errorcluster)  [unwired: 5 in, 1 out]
          }
        }
        n571 = Bundle By Name(cluster=w1577, "Undo Transaction"=FALSE) -> (w1573:T13)
      }
      frame "Script: do undo" {
        n572 = Unbundle By Name(w1587) -> ("CaseStrVI Ref"=w1585:refnum<vi>)
        n573 = invoke class="VI" method="Transaction.Undo"(reference=w1585, error in=w1586) -> (error out=w1589:errorcluster)  [unwired: 1 in, 2 out]
        n574 = call <vilib>:"Clear Errors.vi"("error in (no error)"=w1589) -> ("error out"=w1584:errorcluster)  [unwired: 5 in, 1 out]
      }
      frame "Script: fail undo" {
        n575 = Unbundle By Name(w1595) -> ("CaseStrVI Ref"=w1593:refnum<vi>)
        n576 = Bundle By Name(cluster=w1595, "Undo Transaction"=FALSE) -> (w1591:T13)
        n577 = invoke class="VI" method="Transaction.Fail"(reference=w1593, error in=w1594) -> (error out=w1597:errorcluster)  [unwired: 1 in, 2 out]
        n578 = call <vilib>:"Clear Errors.vi"("error in (no error)"=w1597) -> ("error out"=w1592:errorcluster)  [unwired: 5 in, 1 out]
      }
      frame "Script: append string" {
        w1601 = refnum<vi> refnum  # CaseStructure
        n579 = Unbundle By Name(w1621) -> ("StructRef"=w1600:refnum<vi>, "tag"=w1607:string, "CaseStrVI Ref"=w1619:refnum<vi>)
        n580 = property class="VI"(reference=w1619, error in=w1620) -> (error out=w1616:errorcluster, "Diagram"=w1618:refnum<vi>)  [unwired: 1 out]
        n581 = property class="TopLvlDiag"(reference=w1618, error in=w1616) -> (error out=w1613:errorcluster, "SelList[]"=w1617:refnum<vi>[])  [unwired: 1 out]
        n582 = Search and Replace String(replace all?=TRUE ("replace all? (F)"), input string=w1607, search string="\"") -> (result string=w1608:string)  [unwired: 5 in, 3 out]
        n583 = To More Specific Class(target class=w1601, reference=w1600) -> (specific class reference=w1599:refnum<vi>, error out=w1598:errorcluster)  [unwired: 1 in]
        n584 = call "JKI Arguments Used.vi"("error in"=w1598, "CaseSel Refnum"=w1599) -> ("error out"=w1603:errorcluster, "Arguments used?"=w1604:bool)  [unwired: 8 in]
        n585 = call "RCF Case Select"("Enable"=w1604, "error in (no error)"=w1603) -> ("Argument"=w1602:string)  [unwired: 15 in, 2 out]
        n586 = Array Size(array=w1617) -> (size(s)=w1615:i32)
        n587 = Index Array(array=w1617) -> (element=w1612:refnum<vi>)  [unwired: 1 in]
        n588 = case shown="1" w1615 {
          tunnel: [w1622 w1626] -> w1614
          tunnel: w1613 -> [w1622 w1630]
          tunnel: w1612 -> [_ w1629]
          tunnel: w1608 -> [_ w1624]
          tunnel: w1602 -> [_ w1623]
          frame 0, Default {
          }
          frame 1 {
            w1628 = refnum<vi> refnum  # StringConstant
            n589 = To More Specific Class(target class=w1628, reference=w1629, error in=w1630) -> (specific class reference=w1627:refnum<vi>, error out=w1625:errorcluster)
            n590 = case shown="No Error" w1625 {
              selector: w1625 -> [w1644 w1652]
              tunnel: w1627 -> [w1650 _]
              tunnel: [w1645 w1651] -> w1626
              tunnel: w1624 -> [w1641 _]
              tunnel: w1623 -> [w1633 _]
              frame No Error {
                n591 = property class="StrCnst"(reference=w1650, error in=w1644) -> (reference out=w1646:refnum<vi>, error out=w1649:errorcluster, "Value"=w1640:variant)
                n592 = Empty String/Path?(string/path=w1633) -> (empty?=w1636:bool)
                n593 = Format Into String(format string=" >> %s", w1633) -> (resulting string=w1632:string)  [unwired: 2 in, 1 out]
                n594 = Select(t="", s=w1636, f=w1632) -> (s? t:f=w1631:string)
                n595 = Variant To Data(error in=w1649, type="", Variant=w1640) -> (data=w1642:string, error out=w1647:errorcluster)
                n596 = Format Into String(format string="%s\n%s%s", w1642, w1641, w1631) -> (resulting string=w1638:string)  [unwired: 2 in, 1 out]
                n597 = call <vilib>:"Trim Whitespace.vi"("string"=w1638) -> ("trimmed string"=w1637:string)  [unwired: 1 in]
                n598 = To Variant(anything=w1637) -> (Variant=w1639:variant)
                n599 = property class="StrCnst"(reference=w1646, error in=w1647, "Value"=w1639) -> (error out=w1645:errorcluster)  [unwired: 1 out]
              }
              frame Error {
                # "I don't care..."
                n600 = call <vilib>:"Clear Errors.vi"("error in (no error)"=w1652) -> ("error out"=w1651:errorcluster)  [unwired: 5 in, 1 out]
              }
            }
          }
        }
        n601 = call <vilib>:"Add State(s) to Queue__jki_lib_state_machine.vi"("State(s) in Front (\"\")"="Script: highlight" ("State(s) in Front (\"\")"), "State(s) in (\"\")"=w1611) -> ("States Out"=w1610:string)  [unwired: 13 in]
      }
      frame "Script: highlight" {
        n602 = Unbundle By Name(w1660) -> ("CaseStrVI Ref"=w1656:refnum<vi>)
        n603 = property class="VI"(reference=w1656, error in=w1657) -> (error out=w1658:errorcluster, "Diagram"=w1659:refnum<vi>)  [unwired: 1 out]
        n604 = property class="TopLvlDiag"(reference=w1659, error in=w1658) -> (error out=w1654:errorcluster, "SelList[]"=w1653:refnum<vi>[])  [unwired: 1 out]
        n605 = for {
          tunnel: w1653 -> [w1663] mode=indexing
          shift-right: [w1662] -> w1655
          shift-left: w1654 -> [w1664]
          n606 = invoke class="GObj" method="ObjHighlight"(reference=w1663, error in=w1664) -> (error out=w1662:errorcluster)  [unwired: 1 in, 2 out]
        }
      }
      frame "Script: Mark calling VI Modified" {
        # "32 is the generic 'the VI was recompiled' docmod\nThis will force a dirty dot (*) to appear in the calling VI titlebar and prompt the user to save.\nI fear this is the workaround for a workaround for a bug in LabVIEW."
        n607 = Unbundle By Name(w1669) -> ("CaseStrVI Ref"=w1667:refnum<vi>)
        n608 = invoke class="VI" method="SetVIMod"(reference=w1667, error in=w1668, "Mod"=u64 32) -> (error out=w1665:errorcluster)  [unwired: 1 in, 3 out]
      }
    }
  }
  n609 = flat-sequence {
    tunnel: w11 -> [w1674]
    tunnel: w1 -> [w1672]
    tunnel: w6 -> [w1673]
    frame #0 {
      n610 = call <vilib>:"Simple Error Handler.vi"("error in (no error)"=w1674) -> ()  [unwired: 4 in, 5 out]
      n611 = Close Reference(reference=w1673) -> (error out=w1671:errorcluster)  [unwired: 1 in]
      n612 = Close Reference(reference=w1672, error in (no error)=w1671) -> ()  [unwired: 1 out]
    }
  }
